vi "AlliGator Decay Fit Parameter Map Actions.vi"(0 "AlliGator Q Elements in":T6[](array[typedef]), 1 "VI in":refnum<vi>, 2 "Script in":bool, 5 "data value reference":refnum<data-value>, 7 "AlliGator Q Event in":T7=enum."GUI:Idle", 9 "Data":variant, 11 "error in (no error)":errorcluster) -> (3 "Script out":bool, 4 "AlliGator Q Elements out":T6[](array[typedef]), 6 "Data Value Reference out":refnum<data-value>, 10 "[Notebook Message]":T1[](array[typedef]) {"Message Style"."Font Size" min=6.0 step=1.0}, 15 "error out":errorcluster)   [LabVIEW 2021, in "AlliGator Action Engine.lvlib"]
doc: "Processes AlliGator decay fit parameter map-related actions."
uses:
  AlliGator Action Engine.lvlib
  Internal Variables/AlliGator Internal Variables v2.ctl
  <vilib>/vision/Image Controls.llb/IMAQ Image.ctl
  Internal Variables/AlliGator Gate Image Set.ctl
  Files/AlliGator FLI Dataset Type.ctl
  Files/AlliGator Data Series Type.ctl
  Dual-Channel Datasets/AlliGator Dataset Channel.ctl
  Settings/AlliGator Gate Arithmetic.ctl
  Source Image/AlliGator Displayed Image.ctl
  Image/Named ROI Description.ctl
  Phasor Graph/AlliGator Decay Metadata v3.ctl
  Decay Analysis/Decay Preprocessing/AlliGator Decay Background Subtraction Info.ctl
  Decay Analysis/Decay Preprocessing/AlliGator Baseline Subtraction Method.ctl
  Graphs/XY Graph/XY Graph Plot Shift Parameters.ctl
  Graphs/XY Graph/XY Graph Plot Shift Method.ctl
  Decay Analysis/Decay Preprocessing/AlliGator Decay Extrapolation Parameters.ctl
  Phasor/Calibration Phasor (m, phi).ctl
  Phasor/Phasor Reference Series.ctl
  Phasor/Phasor Calibration Map v2.ctl
  Phasor/Phasor (g, s).ctl
  Phasor Graph/AlliGator Raw Phasor Plot Data v5.ctl
  Phasor/Phasor Standard Deviation Options.ctl
  Phasor Plot/AlliGator Phasor Multi-Harmonic Data.ctl
  Phasor/Phasor Harmonic Data.ctl
  Decay Fit Parameter Map/AlliGator Decay Fit Options & Parameters v4.ctl
  Fits/IRF(X)PSED/Decay Fit Options v4.ctl
  Fits/Decay Convolution/Decay Model.ctl
  Fits/Residual Type.ctl
  Fits/IRF(X)PSED/Fit Weights Type v2.ctl
  Fits/Non-linear Fitting Method v2.ctl
  Fits/Fit Calculation Method.ctl
  Fits/Non-linear Fitting Algorithm.ctl
  Decay Analysis/Decay Fit/AlliGator Decay Fit Parameter Constraints 2.ctl
  Fits/IRF(X)PSED/Decay Fit Parameters In List.ctl
  Fits/IRF(X)PSED/MLE Baseline Offset Type.ctl
  Decay Analysis/Decay Preprocessing/AlliGator Decay Preprocessing Parameters.ctl
  Fits/IRF(X)PSED/Decay Fit Parameters & Derived Quantities List v2.ctl
  Fits/IRF(X)PSED/Decay Fit Result Constraint.ctl
  Decay Fit Parameter Map/AlliGator Parameter Maps Data.ctl
  AlliGator Q Event.ctl
  AlliGator Q Element.ctl
  Notebook/Notebook Message Object.ctl
  Rich Text Box/Text Formatting.ctl
  Rich Text Box/Text Colors.ctl
  Rich Text Box/Text Style.ctl
  Rich Text Box/Text Alignment.ctl
  Alligator Elements Order in Action Stack.ctl
  Globals, Variables, Constants/AlliGator Variables List.ctl
  GUI/AlliGator Image Display Type.ctl
  Palette/Image Palette Information.ctl
  Image/Image Display Palette Type.ctl
  Decay Fit Parameter Map/AlliGator Decay Parameter Map Update Event Data.ctl
  Rich Text Box/Text Format List.ctl
  GUI/AlliGator Windows List.ctl
  Utilities/Read-Write.ctl
  GUI/AlliGator Image Mouse Up Event Data.ctl
  Image/Image ROI Descriptor.ctl
  Image/Image Contour Definition.ctl
  Image/Image Contour ID.ctl
  Image/Image ROI Type.ctl
  Image/Image Control Refnum.ctl
  Files/Load-Save File Info.ctl
  Parameter Map/AlliGator New Parameter Map Set Event Data.ctl
  AlliGator Add Single Action to Stack.vi
  Variant/Variant to Data/Variant to [String].vi
  Variant/Variant to Data/Variant to String.vi
  <userlib>/_OpenG.lib/array/array.llb/Remove Duplicates from 1D Array (String)__ogtk.vi
  Variant/Variant to Data/Variant to I32.vi
  Variant/Variant to Data/Variant to Boolean.vi
  Local Decay Window/AlliGator Local Decay Window.lvlib
  Fits/Fits.lvlib
  Decay Fit Parameter Map/AlliGator Decay Fit Parameter Map.lvlib
  GUI/GUI.lvlib
  Variant/Variant to Data/Variant to Data.lvlib
  Globals, Variables, Constants/AlliGator Globals, Variables & Constants.lvlib
  Palette/Palette.lvlib
  GUI/AlliGator GUI.lvlib
  Image/Image.lvlib
  Files/Files.lvlib
  Sound/Sound.lvlib
  Source Image/AlliGator Source Image+.lvlib
  Parameter Map/AlliGator Parameter Map.lvlib
  Utilities/Utilities.lvlib
  Notebook/Notebook.lvlib
  <userlib>/_OpenG.lib/array/array.llb/openg_array.lvlib
  Phasor/Phasor.lvlib
  Decay Analysis/Decay Preprocessing/AlliGator Decay Preprocessing.lvlib
  Graphs/XY Graph/XY Graph Add-Ons.lvlib
  Phasor Graph/AlliGator Phasor Graph.lvlib
  Files/AlliGator Files.lvlib
  Internal Variables/AlliGator Internal Variables.lvlib
  Phasor Plot/AlliGator Phasor Plot.lvlib
  Decay Analysis/Decay Fit/AlliGator Decay Fit.lvlib
  Settings/AlliGator Settings+.lvlib
  Rich Text Box/Rich Text Box.lvlib
  Dual-Channel Datasets/AlliGator Dual-Channel Datasets.lvlib
panel:
  # "see the License on the block diagram (Ctrl+E or Window:Show Block Diagram)"
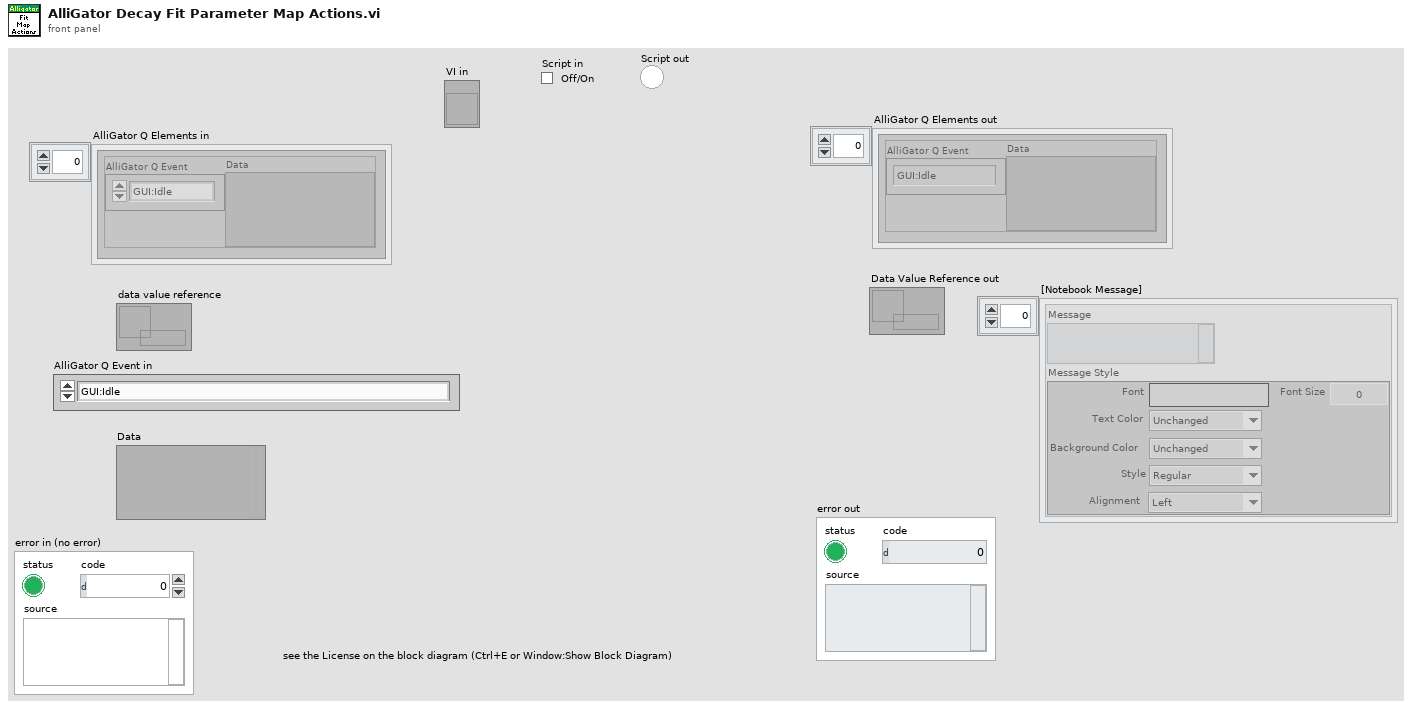
[diagram p1: front panel]
types:
  T1 = typedef "Notebook.lvlib/Notebook Message Object.ctl" = cluster{"Message":string, "Message Style":T2}
  T2 = typedef "Rich Text Box.lvlib/Text Formatting.ctl" = cluster{"Font":string, "Text Color":T3, "Background Color":T3, "Style":T4, "Font Size":dbl, "Alignment":T5}
  T3 = typedef "Rich Text Box.lvlib/Text Colors.ctl" = enum16{"Unchanged", "Black", "Blue", "Cyan", "Maroon", "Gray", "Violet", "Green", "Light Green", "Orange", "Yellow", "Magenta", "Red", "White"}
  T4 = typedef "Rich Text Box.lvlib/Text Style.ctl" = enum16{"Regular", "Bold", "Italic", "Underline", "Strikeout"}
  T5 = typedef "Rich Text Box.lvlib/Text Alignment.ctl" = enum16{"Left", "Right", "Center"}
  T6 = typedef "AlliGator Action Engine.lvlib/AlliGator Q Element.ctl" = cluster{"AlliGator Q Event":T7, "Data":variant}
  T7 = typedef "AlliGator Action Engine.lvlib/AlliGator Q Event.ctl" = enum16{"---- Files ----", "Files:Set Batch Export Files To Save", "Files:Set Dataset Loading & Pre-processing Options", "Files:Check #Frames in Dataset", "Files:Increment Frame Index", "Files:Open Mask Image", "Files:Open White Light Image", "Files:Open Single Dataset", "Files:New Folder of Folders Selected", "Files:Load File (all Types)_Scriptable", "Files:Move Flattened Series to Folders Series", "Files:Select Folder", "Files:Load FLI Dataset", "Files:Load Swiss SPAD 1 Dataset", "Files:Load Swiss SPAD 2 Dataset", "Files:Load .sdt FLI Dataset", "Files:Load .ptu FLI Dataset", "Files:Load .bin FLI Dataset", "Files:Load Single Gate Image Folder", "Files:Load I/m/phi Dataset (deprecated)", "Files:Load Single Image", "Files:Subtract Background File", "Files:Export FLI Dataset", "Files:Load HDF5 FLI Dataset", "Files:Set Destination File Path", "Files:Save Mask Image", "Files:Batch Conversion", "Files:New Folder Selected", "Files:Close FLI Dataset", "Files:Close FLI Dataset Series", "Files:Close White Light Image", "Files:Close Mask Image", "---- FLI Dataset ----", "FLI Dataset:Channel Arithmetic", "FLI Dataset:Export Average Lifetime Map as ASCII", "FLI Dataset:Export User-Defined Quantity Map as ASCII", "FLI Dataset:Python Function FLI Dataset Event", "FLI Dataset:ROI Analysis", "FLI Dataset:Tilted Logistic Square Gated IRF Characteristics Map", "FLI Dataset:Logistic Square Gated IRF Characteristics Map", "FLI Dataset:Square Gated IRF Characteristics Map", "FLI Dataset:Multi-ROI Single-Pixel Phasor Analysis", "FLI Dataset:Multi-ROI Single-Pixel NLSF Analysis", "FLI Dataset:All ROIs IRF Extraction", "FLI Dataset:All ROIs Decay Fit Non-Interactive (Fast + Individual IRF)", "FLI Dataset:All ROIs Phasor Analysis", "FLI Dataset:All ROIs Decay Fit", "FLI Dataset:Fluorescence Decay Statistics", "FLI Dataset:Update Decay Statistics Graph", "FLI Dataset:Get Decay from ROI", "FLI Dataset:All ROIs Average Lifetimes", "FLI Dataset:Save/Load Local IRFs", "FLI Dataset:Clear Local IRFs", "FLI Dataset:Phasor Calibration Maps (# Gates Series) Script", "FLI Dataset:Calibrated Phasor Map Series", "---- FLI Dataset Series ----", "FLI Dataset Series:Sum All Datasets in Series", "FLI Dataset Series:Add Dataset to Accumulated Dataset", "FLI Dataset Series:Display Accumulated Dataset", "FLI Dataset Series:Clear Dataset Series Sum", "FLI Dataset Series:Time-Series Analysis (NLSF)", "FLI Dataset Series:Time-Series Analysis (Phasor)", "---- Image ----", "Image:Update Image Profile Plots", "Image:Image Histogram Cursor Move", "Image:Image Histogram", "Image:Image Contrast", "Image:Set Image Histogram Cursor Move Flag", "Image:Clear Image Overlay", "Image:Use ROI as Search Area", "Image:Set ROI Diameter", "Image:Save Image Data as TIFF", "Image:Save Displayed Image with Overlay", "Image:Save Image Overlay Only", "Image:Save Image as Hot Pixel Mask", "Image:Change Source Image Color Palette", "Image:Copy Image to Clipboard", "Image:Source Image ROI Selection", "Image:Delete All ROIs", "Image:Delete All Unselected ROIs", "Image:Delete ROI", "Image:Merge All ROIs", "Image:Store ROI", "Image:Source Image ROI Storage", "Image:Export ROI Description to Notebook", "Image:Save ROI", "Image:Load ROI", "Image:Paste ROI Definition", "Image:Clear ROI", "Image:Identify ROIs in Mask Image", "Image:Create Complementary ROI", "Image:Create Contour ROI", "Image:Create ROI(s) from Pixels with Peak above Min_Scriptable", "Image:Create ROI(s) from Pixels with Intensity above Min_Scriptable", "Image:Compute ROI Statistics", "Image:Delete ROI(s) based on ROI Characteristics", "Image:Create ROI Grid", "Image:ROI to Individual Pixel ROIs", "Image:Python Function Source Image Event", "Image:Show Phasor Calibration Map ROI Centers", "Image:Convert ROI to Mask Image", "Image:Mouse Move", "Image:Mouse Up", "Image:Set Source Image Mouse Move Flag", "Image:Add Scale Bar Overlay", "Image:Delete Existing ROIs Option", "Image:Overlay ROI Median", "Image:Check Current ROI", "Image:Update True Pixel Value", "Image:Use ROI", "---- Decay ----", "Decay:Clear IRF/Reference Plot", "Decay:Add Decay to Graph", "Decay:Smoothen Plot", "Decay:Smoothen Plot Tail", "Decay:Average Selected Plots", "Decay:Extract IRF", "Decay:Optimal IRF Extraction", "Decay:Threshold IRF", "Decay:Fit to Model IRF", "Decay:Fit IRF to Square Gate", "Decay:Fit IRF to Logistic Square Gate", "Decay:Fit IRF to Tilted Logistic Square Gate", "Decay:Create Bounding Cursors Set", "Decay:Export Bounding Cursors Definition to Notebook", "Decay:Denoise Plot", "Decay:Compute Cumulative Function", "Decay:Use as Reference Decay", "Decay:Show Reference Decay/IRF", "Decay:Extrapolate Decay", "Decay:Create Head & Tail Bounding Cursors", "Decay:Store Cursor-defined Head & Tail Fractions", "Decay:Rebin Plot", "Decay:1-Normalize Decay", "Decay:[0-1]-Normalize Plot", "Decay:Straighten Decay", "Decay:Shift Decay", "Decay:Fold Decay", "Decay:Fit Decay", "Decay:Global Fit of Selected Decays", "Decay:Post Global Fit Script", "Decay:Add Global Fit Parameters to Graph", "Decay:Add Decay Parameter(s) to Plot (Graph)", "Decay:Export Decay to Phasor Graph", "Decay:Compute Average Lifetime", "Decay:Plot Convolution", "Decay:Graph Tip Strip Update", "---- Decay Statistics ----", "Decay Statistics:Tip Strip Update", "---- Intensity Time Trace ----", "Intensity Time Trace:Use File Timestamp", "Intensity Time Trace:Load Intensity Corrections File", "Intensity Time Trace:Clear Intensity Corrections File", "Intensity Time Trace:Tip Strip Update", "---- Phasor Plot ----", "Phasor Plot:Build Phasor Plot", "Phasor Plot:Change Phasor Plot Color Palette", "Phasor Plot:Adjust Phasor Plot Display Range", "Phasor Plot:Highlight Image ROI in Phasor Plot", "Phasor Plot:Save Phasor Plot Image with Overlay", "Phasor Plot:Export Complex Phasor Map", "Phasor Plot:Export Phasor Ratio Map", "Phasor Plot:Export Average Lifetime Map", "Phasor Plot:Compute Phase Lifetime Histogram", "Phasor Plot:Compute Phasor Ratio Histogram", "Phasor Plot:Compute Phase Lifetime vs Intensity Scatter Plot", "Phasor Plot:Weber 2-Component Decomposition", "Phasor Plot:Update Phasor Color Map Vertices", "Phasor Plot:Clear Phasor Overlay", "Phasor Plot:Use Segment Extremities as References", "Phasor Plot:Use UC/Segment Intersections as References", "Phasor Plot:Use UC/Principal Axis Intersections as References", "Phasor Plot:Use UC/Linear Fit Intersections as References", "Phasor Plot:Update Phasor Plot Reference", "Phasor Plot:Show Local Phasor Info in Phasor Plot", "Phasor Plot:Update Phasor Plot State", "Phasor Plot:Phasor Plot ROI Storage", "Phasor Plot:Phasor Plot ROI Selection", "Phasor Plot:Python Function Phasor Plot Event", "Phasor Plot:Overlay Phasor ROI, Ratio or Map in Source Image", "Phasor Plot:Compute Decay of Selected Phasors", "Phasor Plot:Phasor at Image Pixel", "Phasor Plot:Mouse Move", "Phasor Plot:Mouse Up", "Phasor Plot:Display Range Mouse Move", "Phasor Plot:Set Mouse Move Flag", "Phasor Plot:Update True Phasor Plot Value", "---- Phasor Graph ----", "Phasor Graph:Get Phasor Value", "Phasor Graph:Create New Phasor Plot Dialog", "Phasor Graph:Update Last Phasor Value", "Phasor Graph:Update Phasor (m, phi)", "Phasor Graph:Remove Single Phasor from Plot", "Phasor Graph:Add Single Phasor to Plot", "Phasor Graph:Remove Phasor Plot", "Phasor Graph:Remove Selected Phasor Plots", "Phasor Graph:Clear Phasor Data", "Phasor Graph:Clear Phasor Graph", "Phasor Graph:Cursor Move", "Phasor Graph:Draw Cursor Connecting Line", "Phasor Graph:Clear Cursor Connecting Line", "Phasor Graph:Find UC Intersection", "Phasor Graph:Use UC/Cursor-Defined Line Intersections", "Phasor Graph:Use Selected Plots Fitted Line/UC Intersections", "Phasor Graph:Use Selected Plots Principal Axis/UC Intersections", "Phasor Graph:Show Single Phasor", "Phasor Graph:Save Single Phasor Plot", "Phasor Graph:Save All Phasor Plots", "Phasor Graph:Load Phasor Plot(s)", "Phasor Graph:Phasor Multiplication", "Phasor Graph:Compute Average Phasor", "Phasor Graph:Compute Multiple Average Phasors (Selected Plots)", "Phasor Graph:Export Single Phasor Plot Phase Lifetimes", "Phasor Graph:Parameter 2 vs Parameter 1 Scatter Plot", "Phasor Graph:Use Cursor n Location", "Phasor Graph:Set Reference n to Current Phase Lifetime Value", "Phasor Graph:Set Reference n to Lifetime Value", "Phasor Graph:Set Cursor n Location", "Phasor Graph:Save Phasor Graph Image", "Phasor Graph:Update SEPL Plot", "Phasor Graph:Export Single Phasor Plot Data", "Phasor Graph:Export Selected Phasor Plots Data", "Phasor Graph:Python Function Phasor Graph Event", "Phasor Graph:Tip Strip Update", "---- Calibration ----", "Calibration:Set Calibration Type", "Calibration:Load/Save Phasor Calibration", "Calibration:Load/Save Phasor Calibration Series", "Calibration:Load/Save Phasor Calibration Map", "Calibration:Use as Calibration", "Calibration:Compute Optimal Calibration from Phasor References", "Calibration:Clear Phasor Calibration", "Calibration:Single Phasor Calibration Information", "Calibration:Use as Calibration Series", "Calibration:Use as Calibration Map", "Calibration:Clear Calibration Series", "Calibration:Phasor Calibration Series Information", "Calibration:Clear Calibration Map", "Calibration:Phasor Calibration Map Information", "Calibration:Apply Phasor Calibration", "Calibration:Update Single Plot Calibration", "Calibration:Update Multiple Plots Calibration", "Calibration:Clear Single Plot Calibration", "Calibration:Clear All Plots Calibrations", "Calibration:Clear Plot(s) Calibration(s)?", "---- Phasor Ratio ----", "Phasor Ratio:Clear Reference n", "Phasor Ratio:Toggle Selected Plot(s)  Lock to Reference 1", "Phasor Ratio:Use as Reference n", "Phasor Ratio:Send Reference n to Notebook", "Phasor Ratio:Toggle Selected Plot(s)  Lock to Reference 2", "Phasor Ratio:Compute Phasor Ratio at Mouse Location", "Phasor Ratio:Compute Phasor Plot's Average Phasor Ratio", "Phasor Ratio:Compute Time-Series Phasor Ratios", "Phasor Ratio:Fit Line to Phasor Ratio Plot", "Phasor Ratio:Save References", "Phasor Ratio:Load References", "Phasor Ratio:Update Phasor Reference 1", "Phasor Ratio:Update Phasor Reference 2", "Phasor Ratio:Move Cursor n to Reference n", "Phasor Ratio:Use as Phasor Reference 1 Lifetime", "Phasor Ratio:Use as Phasor Reference 2 Lifetime", "Phasor Ratio:Export Phasor Ratio Map as ASCII", "Phasor Ratio:Tip Strip Update", "---- Lifetime & Other Parameters Graph ----", "Lifetime:Compute Sliced Mean, SDV and CV Plots", "Lifetime:Plot Decay Shifts", "Lifetime:Plot Histogram", "---- Decay Fit Parameter Map ----", "Decay Fit Parameter Map:Export ROI NLSF Data as ASCII", "Decay Fit Parameter Map:Set Decay Fit Parameter Map Selection", "Decay Fit Parameter Map:Build Decay Fit Parameter Map", "Decay Fit Parameter Map:Change Decay Fit Parameter Map Color Palette", "Decay Fit Parameter Map:Export Decay Fit Parameter Map Data as ASCII", "Decay Fit Parameter Map:Export All Decay Fit Parameter Maps Data as ASCII", "Decay Fit Parameter Map:Selected Parameter Scatterplot", "Decay Fit Parameter Map:Parameter 2 vs Parameter 1 Scatterplot", "Decay Fit Parameter Map:Save Decay Fit Parameter Map Image", "Decay Fit Parameter Map:Save-Load IRFs & Fit Data", "Decay Fit Parameter Map:Update Local Decay Plots", "Decay Fit Parameter Map:Python Function Decay Fit Parameters Map Event", "Decay Fit Parameter Map:Overlay Decay Fit Parameter Map in Source Image", "Decay Fit Parameter Map:Selected Parameter vs Intensity Scatterplot", "Decay Fit Parameter Map:Mouse Up", "Decay Fit Parameter Map:Mouse Move", "Decay Fit Parameter Map:Display Range Mouse Move", "Decay Fit Parameter Map:Change Map Resolution", "Decay Fit Parameter Map:Variance Significance Maps", "Decay Fit Parameter Map:Fit Result Constraints Window", "Decay Fit Parameter Map:Use ROI", "---- Parameter Map ----", "Parameter Map:Export ROI Parameters Data as ASCII", "Parameter Map:Add Parameter Map Set", "Parameter Map:Delete Parameter Map Set", "Parameter Map:Update Parameter List", "Parameter Map:Build Parameter Map", "Parameter Map:Change Parameter Map Color Palette", "Parameter Map:Export Parameter Map Data as ASCII", "Parameter Map:Export All Parameter Maps Data as ASCII", "Parameter Map:Selected Parameter Scatterplot", "Parameter Map:Parameter 2 vs Parameter 1 Scatterplot", "Parameter Map:Selected Parameter vs Intensity Scatterplot", "Parameter Map:Save Parameter Map Image", "Parameter Map:Save-Load IRFs & Parameter Maps (TODO)", "Parameter Map:Set Parameter Map Selection", "Parameter Map:Python Function Parameter Map Event", "Parameter Map:Overlay Parameter Map in Source Image", "Parameter Map:Update Local Decay Plots", "Parameter Map:Mouse Up", "Parameter Map:Mouse Move", "Parameter Map:Display Range Mouse Move", "Parameter Map:Use ROI", "---- Generic Graph ----", "Generic Graph:Generic XY Graph Event", "Generic Graph:Python Function XY Graph Event", "Generic Graph:New Plot", "Generic Graph:Save Plot", "Generic Graph:XY Plot Histogram", "Generic Graph:Set XY Graph Plot Name", "Generic Graph:Set Last Cursor Style", "Generic Graph:Tip Strip Update", "---- GUI ----", "GUI:Start Script", "GUI:Type of Displayed Image Changed", "GUI:Gate Image Slide Changed", "GUI:Show Busy Icon", "GUI:Show Busy Icon & Abort Button", "GUI:Hide Busy Icon", "GUI:Hide Busy Icon & Abort Button", "GUI:Abort", "GUI:End Script", "GUI:Start Timing", "GUI:End Timing", "GUI:Set State Indicator", "GUI:Send Parameters JSON Strings to Clipboard", "GUI:Set Gate Step", "GUI:Idle", "GUI:Initialization", "GUI:Quit", "GUI:Increment Dataset Index", "GUI:Set Dataset Index to -1", "GUI:Time Series Slider Moved", "GUI:Time Series Slider Changed", "GUI:Toggle Playback or Loop", "GUI:Playback Script", "GUI:Set Phasor Frequency", "GUI:Open Window", "GUI:Start Test Script", "GUI:End Test Script", "GUI:Set Verbose Mode", "GUI:Set Verbose Settings Mode", "GUI:Initialize Python Session", "DEBUG"}
  T8 = typedef "AlliGator Decay Fit Parameter Map.lvlib/AlliGator Decay Fit Parameter Map Control Refnums.ctl" = cluster{"Decay Fit Parameter Map Color Scale":refnum<vi>, "Decay Fit Parameter":refnum<vi>, "Max Parameter":refnum<vi>, "Min Parameter":refnum<vi>, "Decay Fit Parameter Map Display":refnum<vi>, "Decay Fit Parameter Map Display Range":refnum<vi>, "Decay Parameter Map X":refnum<vi>, "Decay Parameter Map Y":refnum<vi>, "Decay Parameter Map Value":refnum<vi>}
  T9 = typedef "AlliGator GUI.lvlib/AlliGator Dataset Ctrl Refnums.ctl" = cluster{"Current Data":refnum<vi>, "Gate Image Slide":refnum<vi>, "Time Point Slide":refnum<vi>, "Current Time Stamp":refnum<vi>, "Save Image":refnum<vi>, "Displayed Image":refnum<vi>, "Phasor Overlay Color":refnum<vi>, "Image Color Scale":refnum<vi>, "Use ROI as Search Area":refnum<vi>, "Source Image ROI Color":refnum<vi>, "True Pixel Value":refnum<vi>, "Source Image Display":refnum<vi>, "CPU":refnum<vi>}
  T10 = typedef "AlliGator Action Engine.lvlib/Alligator Elements Order in Action Stack.ctl" = enum16{"Enqueue 2 AFTER 1", "Enqueue 2 BEFORE 1"}
  T11 = typedef "AlliGator Source Image+.lvlib/AlliGator Image Display Type.ctl" = enum16{"Source Image", "Phasor Plot", "Decay Fit Parameter Map", "Parameter Map"}
  T12 = typedef "AlliGator Globals, Variables & Constants.lvlib/AlliGator Variables List.ctl" = enum16{"---- GUI ----", "GUI:Initialization Status", "GUI:State Indicators Refnum", "GUI:Original AlliGator Menu Items", "GUI:Current Action Loop State", "GUI:Script in progress", "GUI:Playback", "GUI:Loop Playback", "GUI:Search ROI Used", "GUI:Search ROI", "Image Histogram Max Legend Size", "Decay Graph Max Legend Size", "Intensity Graph Max Legend Size", "Decay Statistics Graph Max Legend Size", "Phasor Graph Max Legend Size", "Phasor Ratio Graph Max Legend Size", "Lifetime Graph Max Legend Size", "---- Files ----", "Files:Export Dataset Frames as Individual Files", "Files:Show Batch Export Help Balloons", "Files:Frames in Dataset", "Files:ptu File Frame Start Indices", "Files:Current Frame in Dataset", "Files:Current Frame Timestamp", "Files:Dataset Loaded", "Files:Dataset Metadata", "Files:Dataset Channel", "Files:Dataset Data Description", "Files:Background Dataset Metadata", "Files:Background Dataset Channel", "Files:Background Dataset Data Description", "Files:Background File Subtraction", "Files:Background File Path", "Files:Background File Pile-up Correction", "Files:Background File Pixel Well Capacity", "Files:Background File Scaling Factor", "Files:Current Dataset Load Settings", "Files:Dataset Path", "Files:ICCD-specific Information", "Files:Macrotime Gate Separation", "------ Python Plugins ------", "Python Plugins:Information", "Python Plugins:Python Session", "Python Plugins:Valid Python Session?", "---- Source Image ----", "Source Image:ROIs", "Source Image:Current ROI", "Source Image:ROI Event Refnum", "X_Source Image:Display Range", "X_Source Image:Palette Information", "X_Source Image:Type of Displayed Image", "X_Time Gate Slider", "Source Image:Palette List", "Source Image:Scale", "Source Image:ROI Overlay Color", "Source Image:Overlay to Erase", "Source Image:Is Displayed Image Accumulated", "Source Image:White Light Image Modified", "Source Image:Mask Image Modified", "---- Image Profile Window ----", "Image Profile:Window Event Refnum", "Image Profile:IntensityType", "Image Profile:Intensity Average Type", "Image Profile:Intensity-weighted SDV", "Image Profile:Box Profile Type", "Image Profile:Window Open", "Image Profile:Plotted Fit Parameter", "------ Phasor Graph -------", "Phasor Graph:Show Line", "---- Phasor Plot ---", "Phasor Plot:Parameters Changed", "Phasor Plot:FLI Dataset Modified since last Calculation", "Phasor Harmonics Data", "Selected Phasor Harmonics", "Phasor Harmonic Manager Event Refnum", "Phasor Plot:ROIs", "Phasor Plot:Current ROI", "Phasor Plot:ROI Event Refnum", "Phasor Plot:Image Reference Points", "Phasor Plot:Computed", "Phasor Plot:Palette Information", "Phasor Plot:Palette List", "Phasor Plot:Phasor Ratio Palette Information", "Phasor Plot:Phasor Ratio Palette List", "Phasor Plot:Image Scale", "Phasor Plot:Image Overlay to Erase", "Phasor Plot:Image Elements to Update", "Phasor Plot:Current Calculation Parameters", "Phasor Plot:Current Calibration Options", "Phasor Plot:Reset Cumulated Phasor Plot", "Phasor Plot:Reference 1", "Phasor Plot:Lifetime Reference 1", "Phasor Plot:Reference 1 Frequency", "Phasor Plot:Reference 2", "Phasor Plot:Lifetime Reference 2", "Phasor Plot:Reference 2 Frequency", "---- Decay Analysis ----", "Number of Selected Decays to Fit", "LS Fit Results", "LAR Fit Results", "BS Fit Results", "Last Decay Max - Min", "Best Fit Parameters", "Best Fit Parameter Names", "Actual Size X", "Actual Size Y", "Binning X", "Binning Y", "Actual # Gates", "Dataset Number", "Gates to...", "Gates Skipped", "Gates to keep", "Gate Step", "Gate Separation", "Reversed Gates", "Pile-up Correction", "Pixel Well Capacity", "Background Subtracted", "Background Subtraction Method", "Background Definition Range", "Background File (deprecated)", "Number of Dataset Accumulated", "Array of Accumulated Dataset Paths", "Do Averaged Datasets", "Destination File Path", "Process Plot Target", "Use 1/D as Phasor Frequency", "---- Decay Fit Parameter Map -----", "Decay Fit Parameter Map:Palette Information", "Decay Fit Parameter Map:Palette List", "Decay Fit Parameter Map:X Resolution", "Decay Fit Parameter Map:Y Resolution", "Decay Fit Parameter Map:Use Decay Fit Result Constraints", "Decay Fit Parameter Map:Decay Fit Result Constraints", "Decay Fit Parameter Map:Decay Fit Result Constraints Applied", "---- Parameter Map ----", "Parameter Map:Palette Information", "Parameter Map:Palette List", "------- Local Decay Window ---------", "Local Decay Graph Window:Event Refnum", "Local Decay Graph Window:Use normalized IRF for convolution", "----- Miscellaneous ----", "Misc:Skippable Dialog Windows Status"}
  T13 = typedef "Palette.lvlib/Image Palette Information.ctl" = cluster{"Palette Name [# Colors,int?,inv?]":string, "Palette Type":T14, "Palette Colors":u32[], "Interpolate?":bool}
  T14 = typedef "Image.lvlib/Image Display Palette Type.ctl" = u32
  T15 = typedef "Notebook.lvlib/Text Format List.ctl" = enum16{"Message", "Result", "Error", "Setting", "Verbose", "Warning"}
  T16 = typedef "AlliGator Decay Fit Parameter Map.lvlib/AlliGator Decay Parameter Map Update Event Data.ctl" = cluster{"Parameter":T17, "Parameter changed":bool}
  T17 = typedef "Fits.lvlib/Decay Fit Parameters & Derived Quantities List v2.ctl" = enum16{"Offset", "Baseline", "A_1", "tau_1", "A_2", "tau_2", "<tau>_a", "f1_a", "f2_a", "<tau>_i", "f1_i", "f2_i", "-", "R^2", "Chi^2"}
  T18 = typedef "AlliGator GUI.lvlib/AlliGator Windows List.ctl" = enum16{"AlliGator Window", "Settings Window", "Notebook Window", "Dataset Information Window", "Source Image ROI Manager Window", "Phasor Plot ROI Manager Window", "Phasor Harmonic Manager Window", "Histogram Window", "Image Profile Window", "Local Decay Window", "About Window", "Batch Conversion Window", "Shot Noise Influence on Average Lifetime", "Fit Method Benchmark", "Camera Noise Influence on Lifetime", "AlliGator Alias Definition", "Fit Result Constraints Window"}
  T19 = typedef "Utilities.lvlib/Read-Write.ctl" = enum16{"Read", "Write"}
  T20 = typedef "AlliGator GUI.lvlib/AlliGator Image Mouse Up Event Data.ctl" = cluster{"Current ROI Tool":u32, "ROI Descriptor":T21, "Shift":bool, "Alt":bool, "Image Display Refnum":T25}
  T21 = typedef "Image.lvlib/Image ROI Descriptor.ctl" = cluster{"Global Rectangle":i32[], "Contours":T22[]}
  T22 = typedef "Image.lvlib/Image Contour Definition.ctl" = cluster{"Contour Type":T23, "ROI Type":T24, "Points":i32[]}
  T23 = typedef "Image.lvlib/Image Contour ID.ctl" = enum32{"External", "Internal"}
  T24 = typedef "Image.lvlib/Image ROI Type.ctl" = enum16{"No Selection", "Point", "Line", "Rectangle", "Oval", "Polygon", "Freehand Region", "Annulus", "Unused2", "Unused3", "Broken Line", "Freehand Line", "Rotated Rectangle"}
  T25 = typedef "Image.lvlib/Image Control Refnum.ctl" = refnum<vi>
  T26 = cluster{"Fit Parameter 1":T17, "Fit Parameter 2":T17}
  T27 = typedef "Files.lvlib/Load-Save File Info.ctl" = cluster{"Load/Save":bool, "File Path":path}
  T28 = typedef "AlliGator Parameter Map.lvlib/AlliGator New Parameter Map Set Event Data.ctl" = cluster{"New Parameter Set Name":string, "Parameter Map Names":string[]}
  T29 = typedef "Fits.lvlib/Decay Fit Parameters & Derived Quantities List.ctl" = enum16{"Offset", "Baseline", "A_1", "tau_1", "A_2", "tau_2", "<tau>_a", "f1_a", "f2_a", "<tau>_i", "f1_i", "f2_i", "-", "R^2", "Chi^2"}
  T30 = typedef "ROI Descriptor" = cluster{"Global Rectangle":i32[], "Contours":cluster{"ID":enum32{"External", "Internal"}, "Type":u32, "Coordinates":i32[]}[]}
  T31 = typedef "AlliGator Decay Fit Parameter Map.lvlib/AlliGator Function Parameters.ctl" = cluster{"Function":T32, "Amplitude":dbl, "Exponent/Scale":dbl, "Baseline":dbl, "Residuals SDV":dbl, "Minimum CL (%)":dbl, "Analysis Type":enum32{"Reference", "New Sample"}, "Bootstrap SDV x Scale Factor":dbl, "Residuals SDV x Scale Factor":dbl, "Low CL Percentile to Reject (%)":dbl}
  T32 = typedef "AlliGator Lifetime & Other Parameters.lvlib/AlliGator CV(tau) Model Function.ctl" = enum16{"Single-Exponential", "Power Law"}
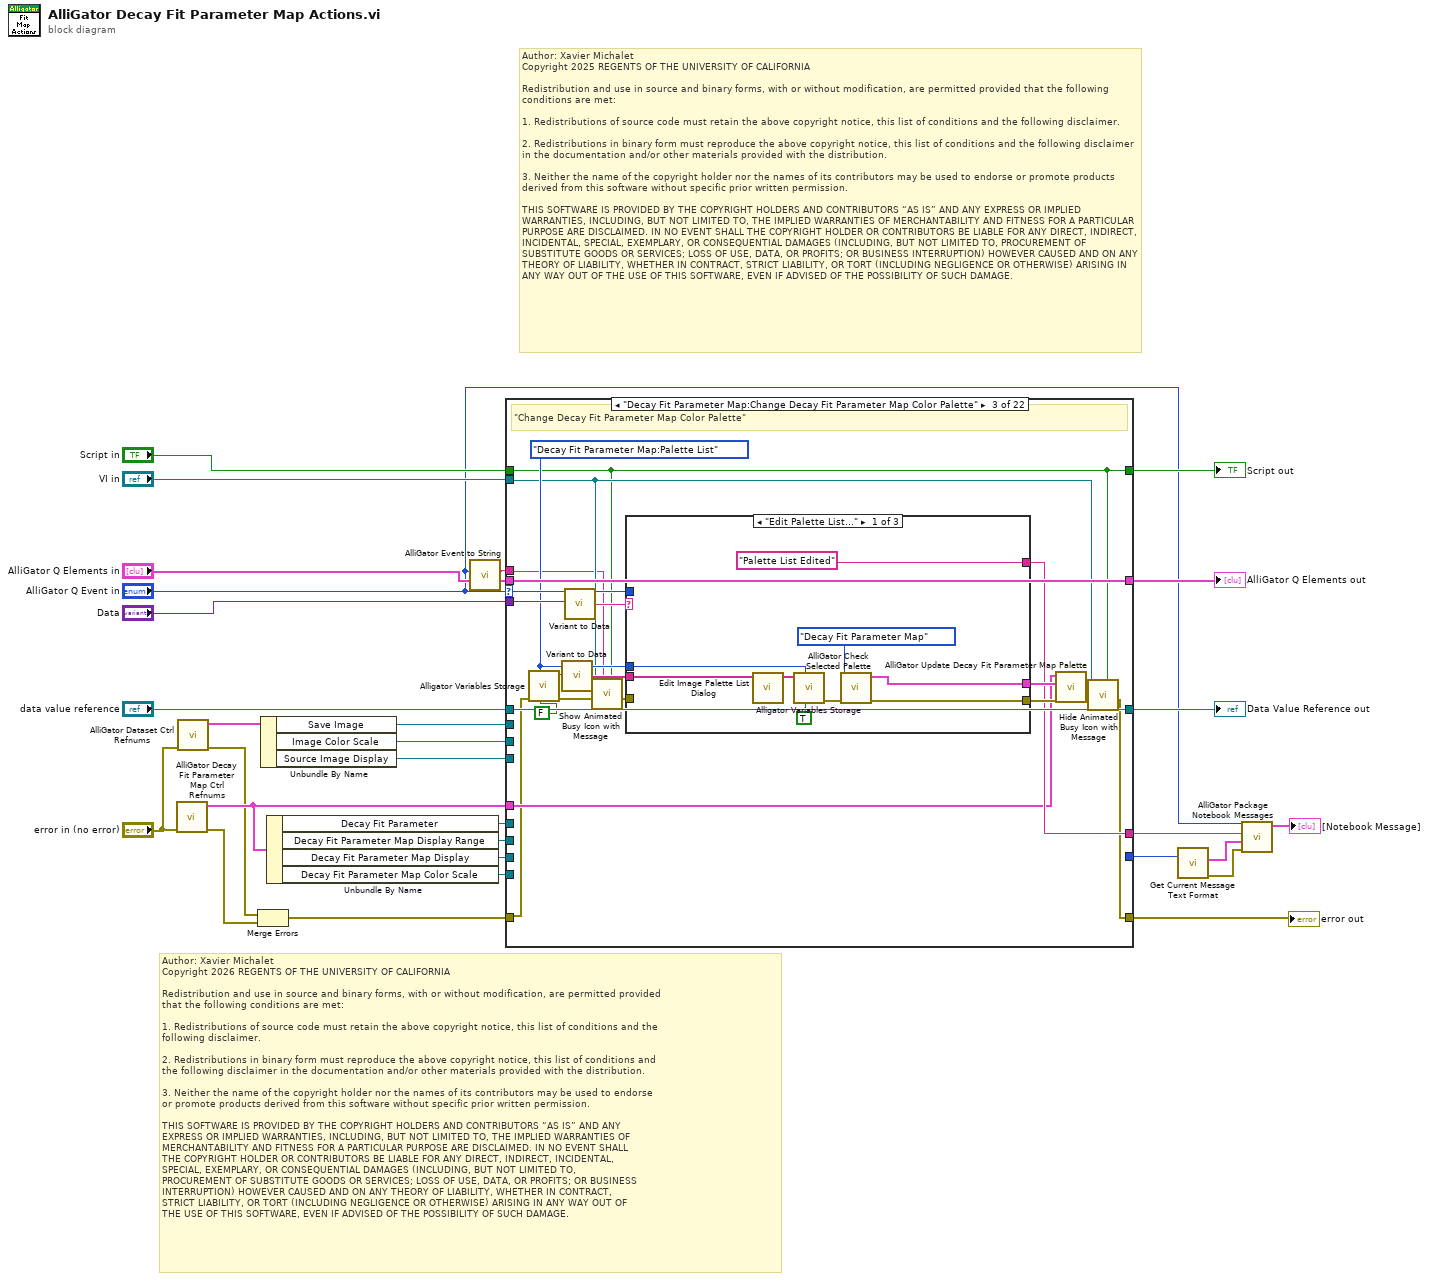
[diagram p0: block diagram]
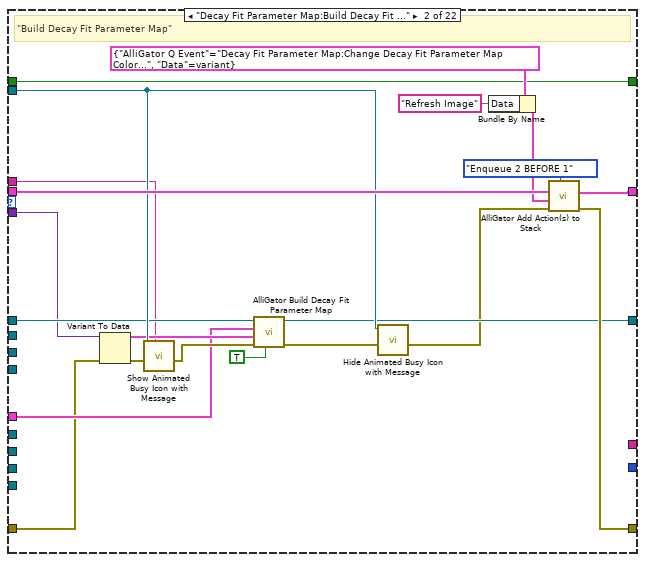
[diagram p3: hidden frame]
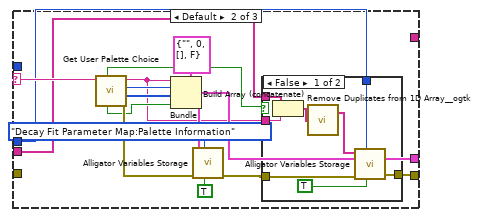
[diagram p4: hidden frame]
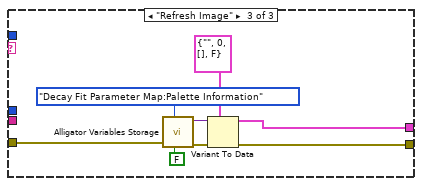
[diagram p6: hidden frame]
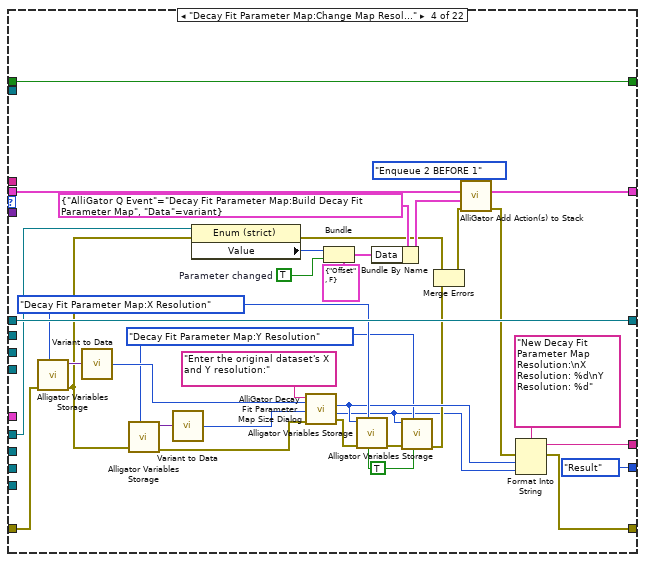
[diagram p7: hidden frame]
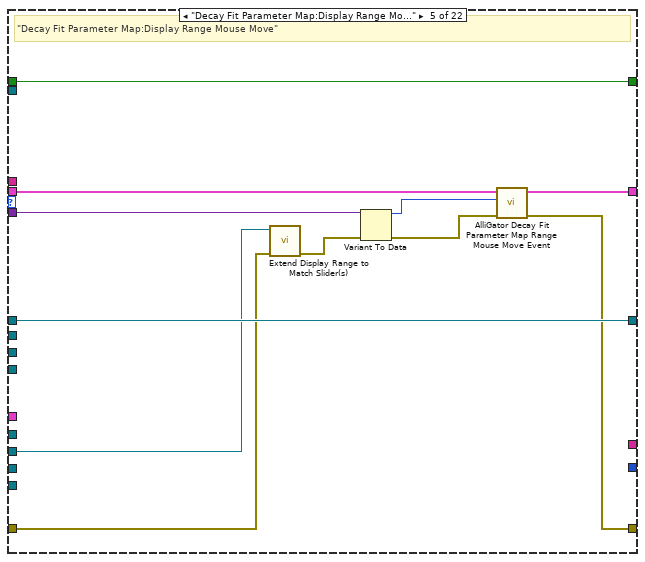
[diagram p8: hidden frame]
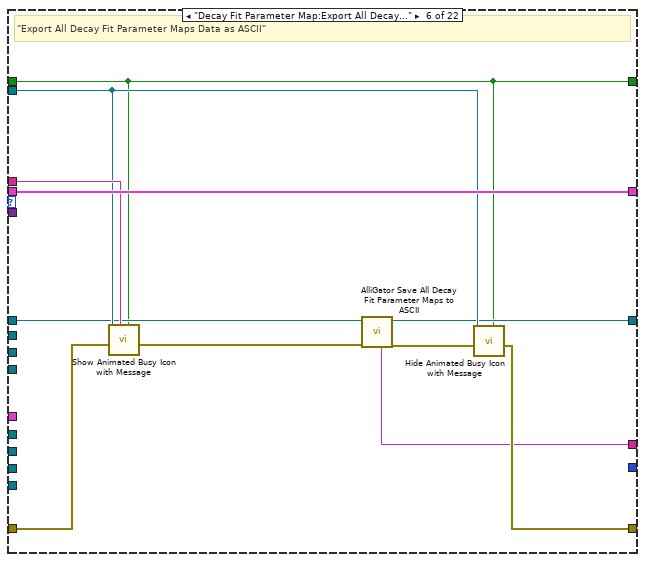
[diagram p9: hidden frame]
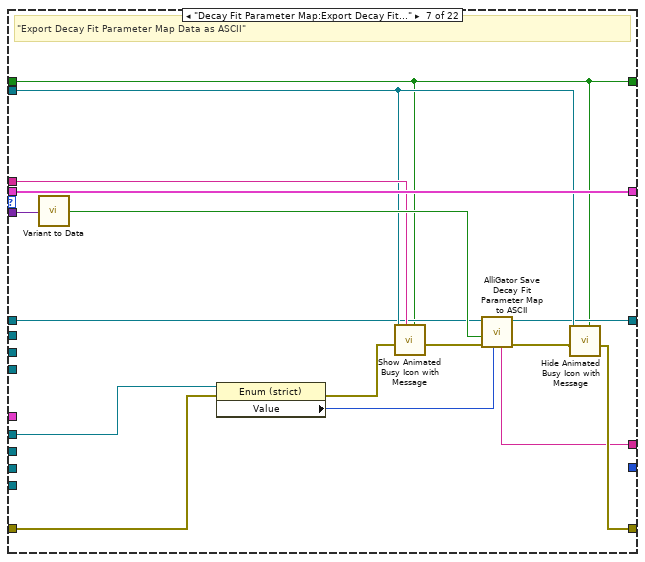
[diagram p10: hidden frame]
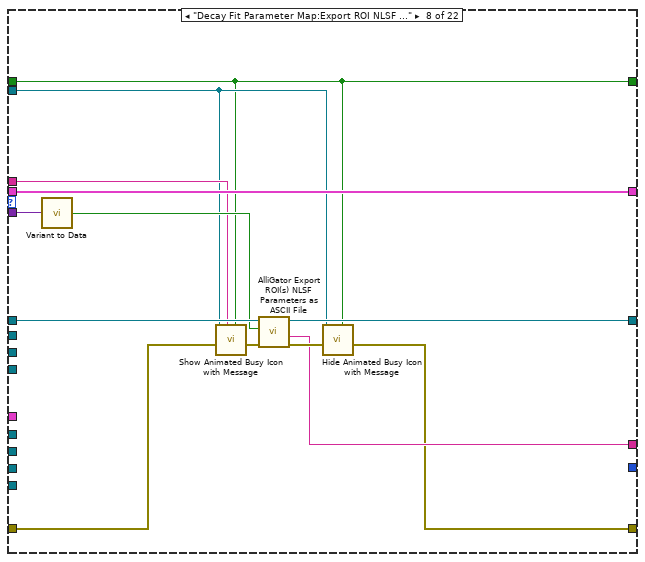
[diagram p11: hidden frame]
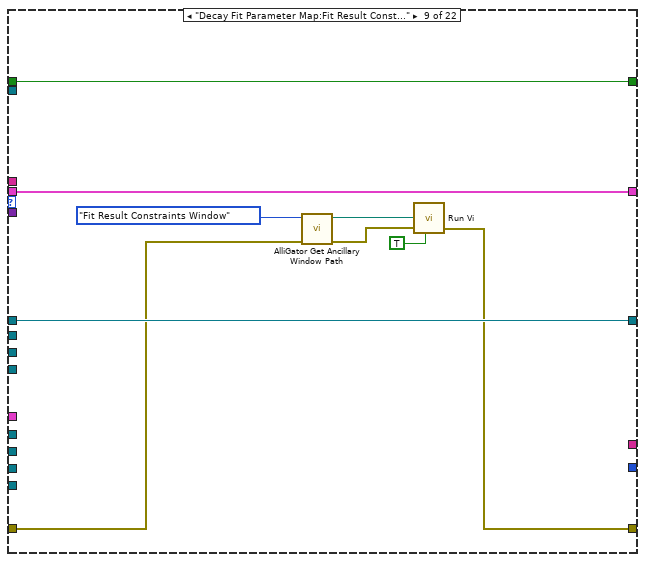
[diagram p12: hidden frame]
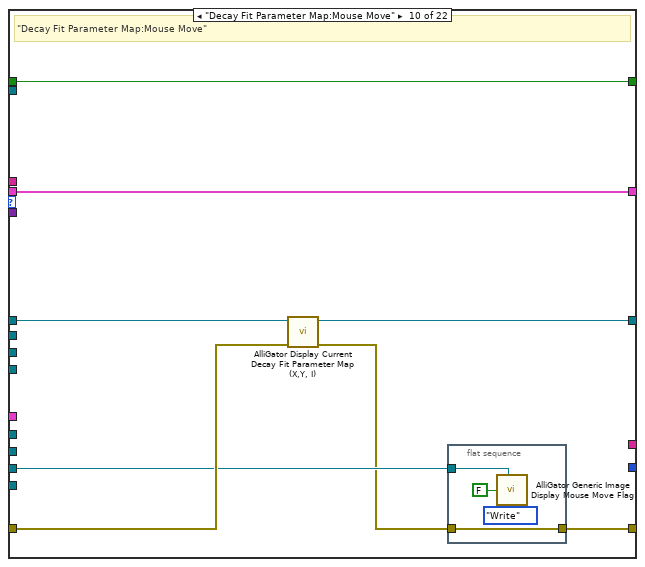
[diagram p13: hidden frame]
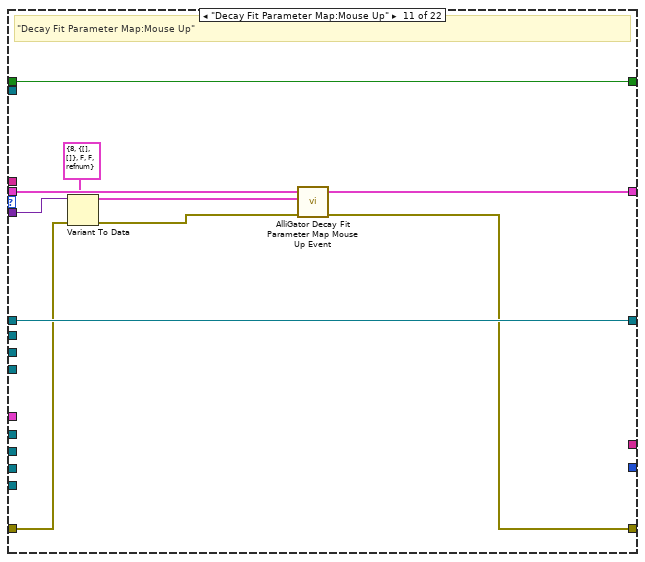
[diagram p14: hidden frame]
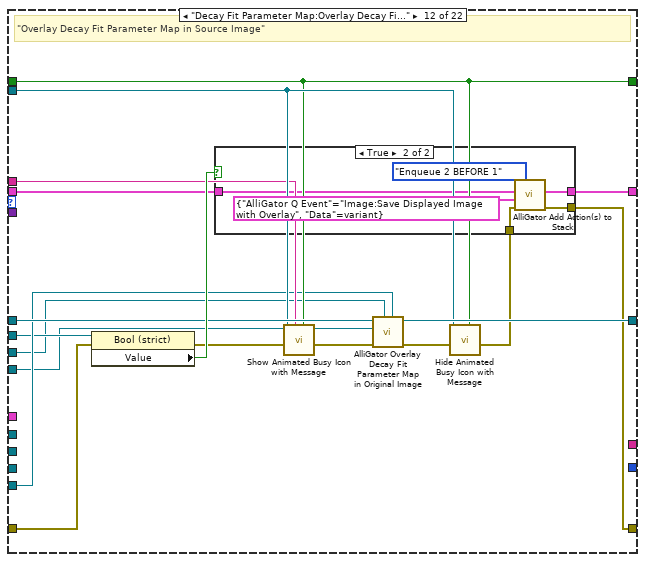
[diagram p15: hidden frame]
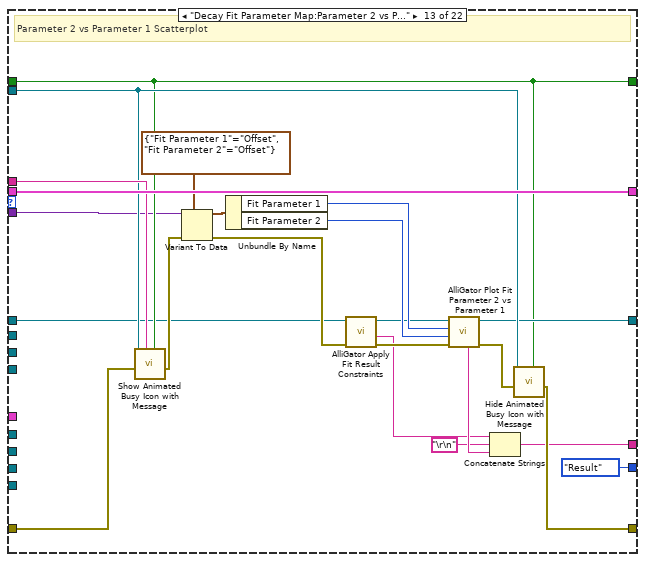
[diagram p17: hidden frame]
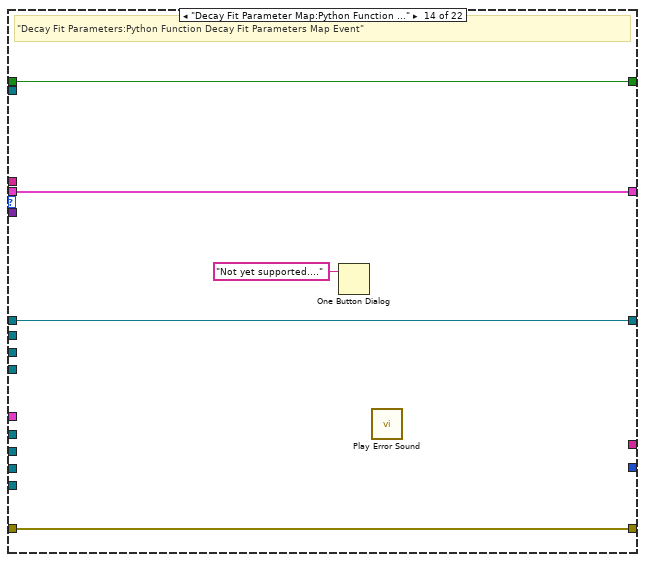
[diagram p18: hidden frame]
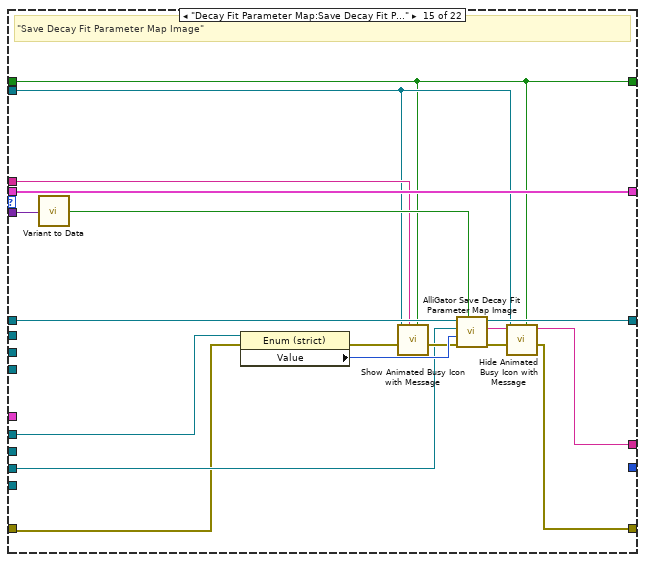
[diagram p19: hidden frame]
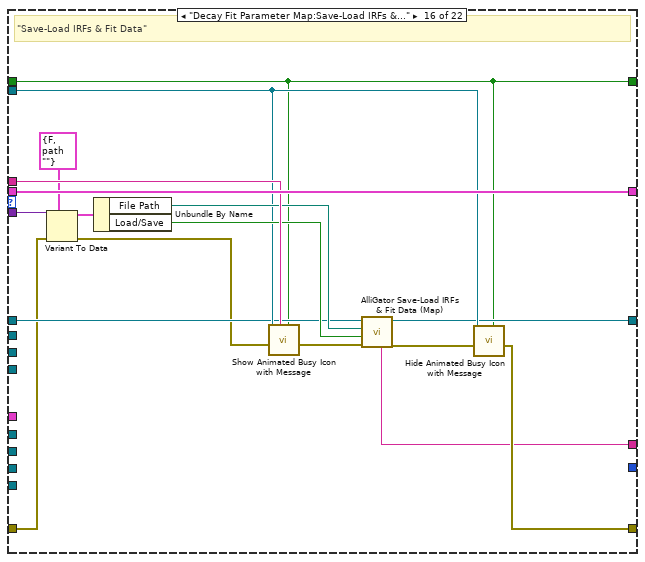
[diagram p20: hidden frame]
diagram:
  # "Author: Xavier Michalet\nCopyright 2026 REGENTS OF THE UNIVERSITY OF CALIFORNIA\n\nRedistribution and use in source and binary forms, with or without modification, are permitted provided\nthat the following conditions are met:\n\n1. Redistributions of source code must retain the above copyright notice, this list of conditions and the\nfollowing disclaimer.\n\n2. Redistributions in binary form must reproduce the above copyright notice, this list of conditions and\nthe following disclaimer in the documentation and/or other materials provided with the distribution.\n\n3. Neither the name of the copyright holder nor the names of its contributors may be used to endorse \nor promote products derived from this software without specific prior written permission.\n\nTHIS SOFTWARE IS PROVIDED BY THE COPYRIGHT HOLDERS AND CONTRIBUTORS “AS IS” AND ANY \nEXPRESS OR IMPLIED WARRANTIES, INCLUDING, BUT NOT LIMITED TO, THE IMPLIED WARRANTIES OF\nMERCHANTABILITY AND FITNESS FOR A PARTICULAR PURPOSE ARE DISCLAIMED. IN NO EVENT SHALL\nTHE COPYRIGHT HOLDER OR CONTRIBUTORS BE LIABLE FOR ANY DIRECT, INDIRECT, INCIDENTAL, \nSPECIAL, EXEMPLARY, OR CONSEQUENTIAL DAMAGES (INCLUDING, BUT NOT LIMITED TO, \nPROCUREMENT OF SUBSTITUTE GOODS OR SERVICES; LOSS OF USE, DATA, OR PROFITS; OR BUSINESS\nINTERRUPTION) HOWEVER CAUSED AND ON ANY THEORY OF LIABILITY, WHETHER IN CONTRACT, \nSTRICT LIABILITY, OR TORT (INCLUDING NEGLIGENCE OR OTHERWISE) ARISING IN ANY WAY OUT OF\nTHE USE OF THIS SOFTWARE, EVEN IF ADVISED OF THE POSSIBILITY OF SUCH DAMAGE."
  # "Author: Xavier Michalet\nCopyright 2025 REGENTS OF THE UNIVERSITY OF CALIFORNIA\n\nRedistribution and use in source and binary forms, with or without modification, are permitted provided that the following conditions are met:\n\n1. Redistributions of source code must retain the above copyright notice, this list of conditions and the following disclaimer.\n\n2. Redistributions in binary form must reproduce the above copyright notice, this list of conditions and the following disclaimer in the documentation and/or other materials provided with the distribution.\n\n3. Neither the name of the copyright holder nor the names of its contributors may be used to endorse or promote products derived from this software without specific prior written permission.\n\nTHIS SOFTWARE IS PROVIDED BY THE COPYRIGHT HOLDERS AND CONTRIBUTORS “AS IS” AND ANY EXPRESS OR IMPLIED WARRANTIES, INCLUDING, BUT NOT LIMITED TO, THE IMPLIED WARRANTIES OF MERCHANTABILITY AND FITNESS FOR A PARTICULAR PURPOSE ARE DISCLAIMED. IN NO EVENT SHALL THE COPYRIGHT HOLDER OR CONTRIBUTORS BE LIABLE FOR ANY DIRECT, INDIRECT, INCIDENTAL, SPECIAL, EXEMPLARY, OR CONSEQUENTIAL DAMAGES (INCLUDING, BUT NOT LIMITED TO, PROCUREMENT OF SUBSTITUTE GOODS OR SERVICES; LOSS OF USE, DATA, OR PROFITS; OR BUSINESS INTERRUPTION) HOWEVER CAUSED AND ON ANY THEORY OF LIABILITY, WHETHER IN CONTRACT, STRICT LIABILITY, OR TORT (INCLUDING NEGLIGENCE OR OTHERWISE) ARISING IN ANY WAY OUT OF THE USE OF THIS SOFTWARE, EVEN IF ADVISED OF THE POSSIBILITY OF SUCH DAMAGE."
  n1 = call "AlliGator Decay Fit Parameter Map Ctrl Refnums.vi"("error in (no error)"="error in (no error)") -> ("error out"=w1:errorcluster, "Decay Fit Map Ctrl Refums"=w13:T8)  [unwired: 9 in]
  n2 = call "AlliGator Dataset Ctrl Refnums.vi"("error in (no error)"="error in (no error)") -> ("error out"=w3:errorcluster, "Dataset Control References"=w8:T9)  [unwired: 9 in]
  n3 = Merge Errors(w3, w1) -> (w2:errorcluster)
  n4 = Unbundle By Name(w8) -> ("Save Image"=w7:refnum<vi>, "Image Color Scale"=w6:refnum<vi>, "Source Image Display"=w5:refnum<vi>)
  n5 = Unbundle By Name(w13) -> ("Decay Fit Parameter"=w12:refnum<vi>, "Decay Fit Parameter Map Display Range"=w11:refnum<vi>, "Decay Fit Parameter Map Display"=w10:refnum<vi>, "Decay Fit Parameter Map Color Scale"=w9:refnum<vi>)
  n6 = call "AlliGator Event to String.vi"("AlliGator Q Event"="AlliGator Q Event in") -> ("String"=w22:string)  [unwired: 8 in]
  n7 = case shown="\"Decay Fit Parameter Map:Change Decay Fit Parameter Map Color Palette\"" "AlliGator Q Event in" {
    selector: "AlliGator Q Event in" -> [_ _ w74 _ _ _ _ _ _ _ _ _ _ _ _ _ _ _ _ _ _ _]
    tunnel: "Data" -> [_ w40 w75 _ w157 _ w188 w201 _ _ w228 _ w275 _ w303 w318 w339 w361 w376 w389 _ w434]
    tunnel: "AlliGator Q Elements in" -> [w33 w54 w71 w142 w160 w173 w189 w202 w211 w219 w231 w246 w282 w287 w304 w321 w342 w364 w377 w390 w404 w439]
    tunnel: [w33 w53 w71 w141 w159 w173 w189 w202 w211 w219 w230 w245 w282 w287 w304 w321 w342 w364 w377 w390 w403 w439] -> w24
    tunnel: "VI in" -> [_ w45 w59 _ _ w170 w183 w192 _ _ _ w244 w279 _ w292 w313 w337 w359 _ w381 w394 _]
    tunnel: "Script in" -> [w30 w37 w58 w150 w161 w165 w178 w191 w209 w218 w232 w243 w276 w283 w291 w308 w333 w355 w367 w380 w393 w437]
    tunnel: w22 -> [_ w38 w57 _ _ w171 w185 w194 _ _ _ w242 w280 _ w294 w319 w340 w362 _ w379 w392 _]
    tunnel: w2 -> [w32 w34 w55 w143 w154 w163 w174 w190 w204 w217 w224 w236 w260 w286 w288 w305 _ w343 w365 w378 w396 w433]
    tunnel: [w32 w47 w60 w132 w158 w172 w186 w193 w203 w212 w229 w239 w281 w286 w293 w320 w341 w363 w368 w382 w395 w432] -> w14
    tunnel: "data value reference" -> [w31 w44 w69 w151 w162 w168 w181 w200 w210 w216 w233 w248 w266 w285 w302 w311 w329 w352 w370 w387 w405 w438]
    tunnel: [w31 w43 w69 w151 w162 w169 w182 w199 w210 w215 w233 w247 w278 w285 w301 w312 w335 w357 w370 w386 w401 w438] -> w29
    tunnel: [_ _ w67 w130 _ w164 w177 w196 _ _ _ _ w264 _ w300 w307 w326 w348 w369 _ w402 _] -> w19
    tunnel: [w30 w37 w58 w150 w161 w165 w178 w191 w209 w218 w232 w243 w276 w283 w291 w308 w333 w355 w367 w380 w393 w437] -> w21
    tunnel: [_ _ _ Text_Format_List."Result" ("Text Format") _ _ _ _ _ _ _ _ Text_Format_List."Result" ("Text Format") _ _ _ Text_Format_List."Result" ("Text Format") Text_Format_List."Result" ("Text Format") _ _ Text_Format_List."Result" ("Text Format") _] -> w16
    tunnel: w13 -> [_ w35 w56 _ _ _ _ _ _ _ _ _ _ _ _ _ _ _ _ _ _ _]
    tunnel: w12 -> [_ _ _ w120 _ _ w175 _ _ _ _ _ _ _ w289 _ w322 w344 w366 _ w391 _]
    tunnel: w11 -> [_ _ _ _ w152 _ _ _ _ _ _ _ _ _ _ _ _ _ _ _ _ _]
    tunnel: w10 -> [_ _ _ _ _ _ _ _ _ w214 _ _ _ _ w290 _ _ _ _ _ _ w430]
    tunnel: w9 -> [_ _ _ _ _ _ _ _ _ _ _ w238 _ _ _ _ _ _ _ _ _ _]
    tunnel: w7 -> [_ _ _ _ _ _ _ _ _ _ _ w237 _ _ _ _ _ _ _ _ _ _]
    tunnel: w6 -> [_ _ _ _ _ _ _ _ _ _ _ w235 _ _ _ _ _ _ _ _ _ _]
    tunnel: w5 -> [_ _ _ _ _ _ _ _ _ _ _ w234 _ _ _ _ _ _ _ _ _ _]
    frame "---- Decay Fit Parameter Map ----", Default {
    }
    frame "Decay Fit Parameter Map:Build Decay Fit Parameter Map" {
      # "\"Build Decay Fit Parameter Map\""
      n8 = Variant To Data(error in=w34, Variant=w40) -> (data=w41:T16, error out=w39:errorcluster)  [unwired: 1 in]
      n9 = call "Show Animated Busy Icon with Message.vi"("Message"=w38, "Error In"=w39, "Target VI Refnum"=w45) -> ("Error Out"=w46:errorcluster)  [unwired: 8 in]
      n10 = call "AlliGator Build Decay Fit Parameter Map.vi"("Compute Decay Fit Parameter Map (T)"=TRUE, "error in (no error)"=w46, "Decay Fit Parameter Map Update Event Data"=w41, "Decay Fit Map Ctrl Refums"=w35, "AlliGator Internal Variables DVR"=w44) -> ("error out"=w52:errorcluster, "AlliGator Internal Variables DVR"=w43:refnum<data-value>)  [unwired: 1 in, 4 out]
      n11 = call "Hide Animated Busy Icon with Message.vi"("Error In"=w52, "Target VI reference"=w45) -> ("Error Out"=w42:errorcluster)  [unwired: 9 in]
      n12 = Bundle By Name(cluster=T6 {"AlliGator Q Event"=enum."Decay Fit Parameter Map:Change Decay Fit Parameter Map Color Palette", "Data"=variant} ("Alligator Atomic Action"), "Data"="Refresh Image") -> (w48:T6)
      n13 = call-poly "AlliGator Add Action(s) to Stack.vi"("Elements Order in Action Stack (Default: 2 BEFORE 1)"=Alligator_Elements_Order_in_Action_Stack."Enqueue 2 BEFORE 1", "Error In"=w42, "Alligator Atomic Action"=w48, "Alligator Queue Element 1"=w54) -> ("Error Out"=w47:errorcluster, "Alligator Queue Element 1 (+ 2)"=w53:T6[])  [unwired: 6 in]
    }
    frame "Decay Fit Parameter Map:Change Decay Fit Parameter Map Color Palette" {
      w63 = AlliGator_Variables_List."Decay Fit Parameter Map:Palette List" ("Alligator Variable")
      # "\"Change Decay Fit Parameter Map Color Palette\""
      n14 = call "Alligator Variables Storage.vi"("Get(F)/Set"=FALSE, "AlliGator Variable"=w63, "Error In"=w55) -> ("Error Out"=w62:errorcluster, "Data out"=w66:variant)  [unwired: 6 in, 1 out]
      n15 = call-poly "Variant to Data.vi"("Variant"=w66) -> ("String Array"=w64:string[])  [unwired: 8 in]
      n16 = call-poly "Variant to Data.vi"("Variant"=w75) -> ("String"=w73:string)  [unwired: 8 in]
      n17 = call "Show Animated Busy Icon with Message.vi"("Already active? (F)"=w58, "Message"=w57, "Error In"=w62, "Target VI Refnum"=w59) -> ("Error Out"=w61:errorcluster)  [unwired: 7 in]
      n18 = case shown="\"Edit Palette List...\"" w73 {
        selector: w73 -> [_ w99 _]
        tunnel: w74 -> [_ _ _]
        tunnel: [w81 w86 w113] -> w72
        tunnel: [w80 w92 w111] -> w70
        tunnel: ["Palette List Edited" ("Append to Message") _ _] -> w67
        tunnel: w64 -> [w77 w90 _]
        tunnel: w63 -> [w76 w85 _]
        tunnel: w61 -> [_ _ w109]
        frame "Edit Palette List..." {
          n19 = call "Edit Image Palette List Dialog.vi"("Palette List (in)"=w77) -> ("Palette List (out)"=w84:string[])  [unwired: 10 in]
          n20 = call "Alligator Variables Storage.vi"("Get(F)/Set"=TRUE, "AlliGator Variable"=w76, "Data in"=w84) -> ("Error Out"=w82:errorcluster)  [unwired: 6 in, 2 out]
          n21 = call "AlliGator Check Selected Palette.vi"("Error In"=w82, "Image"=AlliGator_Image_Display_Type."Decay Fit Parameter Map") -> ("Error Out"=w81:errorcluster, "Image Display Palette Information"=w80:T13)  [unwired: 8 in]
        }
        frame Default {
          n22 = call "Get User Palette Choice.vi"("Palette"=w99) -> ("Error Out"=w95:errorcluster, "Palette Colors"=w97:u32[], "Palette Type"=w98:T14, "Palette Name (# Colors)"=w88:string, "Interpolate?"=w93:bool, "Built-in Palette?"=w89:bool)  [unwired: 3 in, 2 out]
          n23 = Bundle(cluster=T13 {"Palette Name [# Colors,int?,inv?]"="", "Palette Type"=0, "Palette Colors"=[], "Interpolate?"=FALSE} ("Image Display Palette Information"), "Palette Name [# Colors,int?,inv?]"=w88, "Palette Type"=w98, "Palette Colors"=w97, "Interpolate?"=w93) -> (w92:T13)
          n24 = call "Alligator Variables Storage.vi"("Get(F)/Set"=TRUE, "AlliGator Variable"=AlliGator_Variables_List."Decay Fit Parameter Map:Palette Information" ("Alligator Variable"), "Error In"=w95, "Data in"=w92) -> ("Error Out"=w87:errorcluster)  [unwired: 5 in, 2 out]
          n25 = case shown="False" w89 {
            tunnel: w87 -> [w107 w108]
            tunnel: [w106 w108] -> w86
            tunnel: w88 -> [w105 _]
            tunnel: w90 -> [w104 _]
            tunnel: w85 -> [w100 _]
            frame False {
              n26 = Build Array (concatenate)(w104, w105) -> (w103:string[])
              n27 = call-poly <userlib>:"Remove Duplicates from 1D Array__ogtk.vi"("Input Array"=w103) -> ("Output Array"=w102:string[])  [unwired: 1 out]
              n28 = call "Alligator Variables Storage.vi"("Get(F)/Set"=TRUE, "AlliGator Variable"=w100, "Error In"=w107, "Data in"=w102) -> ("Error Out"=w106:errorcluster)  [unwired: 5 in, 2 out]
            }
            frame True {
            }
          }
        }
        frame "Refresh Image" {
          n29 = call "Alligator Variables Storage.vi"("Get(F)/Set"=FALSE, "AlliGator Variable"=AlliGator_Variables_List."Decay Fit Parameter Map:Palette Information" ("Alligator Variable"), "Error In"=w109) -> ("Error Out"=w114:errorcluster, "Data out"=w115:variant)  [unwired: 6 in, 1 out]
          n30 = Variant To Data(error in=w114, type=T13 {"Palette Name [# Colors,int?,inv?]"="", "Palette Type"=0, "Palette Colors"=[], "Interpolate?"=FALSE} ("Image Display Palette Information"), Variant=w115) -> (data=w111:T13, error out=w113:errorcluster)
        }
      }
      n31 = call "AlliGator Update Decay Fit Parameter Map Palette.vi"("error in (no error)"=w72, "Decay Fit Parameter Map Display Palette Information"=w70, "Decay Fit Map Ctrl Refums"=w56) -> ("error out"=w68:errorcluster)  [unwired: 8 in]
      n32 = call "Hide Animated Busy Icon with Message.vi"("Already active? (F)"=w58, "Error In"=w68, "Target VI reference"=w59) -> ("Error Out"=w60:errorcluster)  [unwired: 8 in]
    }
    frame "Decay Fit Parameter Map:Change Map Resolution" {
      w125 = TRUE ("Get(F)/Set")
      w138 = TRUE  # Parameter changed
      w124 = AlliGator_Variables_List."Decay Fit Parameter Map:Y Resolution" ("Alligator Variable")
      w128 = AlliGator_Variables_List."Decay Fit Parameter Map:X Resolution" ("Alligator Variable")
      n33 = call "Alligator Variables Storage.vi"("AlliGator Variable"=w128, "Error In"=w143) -> ("Error Out"=w119:errorcluster, "Data out"=w147:variant)  [unwired: 7 in, 1 out]
      n34 = call-poly "Variant to Data.vi"("Variant"=w147) -> ("Value"=w146:i32)  [unwired: 8 in]
      n35 = call "Alligator Variables Storage.vi"("AlliGator Variable"=w124, "Error In"=w119) -> ("Error Out"=w144:errorcluster, "Data out"=w148:variant)  [unwired: 7 in, 1 out]
      n36 = call-poly "Variant to Data.vi"("Variant"=w148) -> ("Value"=w145:i32)  [unwired: 8 in]
      n37 = property class="Enum (strict)"(reference=w120, error in=w119) -> (error out=w117:errorcluster, "Value"=w134:T17)  [unwired: 1 out]
      n38 = call "AlliGator Decay Fit Parameter Map Size Dialog.vi"("error in (no error)"=w144, "Y Resolution"=w145, "X Resolution"=w146, "Message"="Enter the original dataset's X and Y resolution:") -> ("error out"=w129:errorcluster, "Y Resolution"=w122:i32, "X Resolution"=w127:i32)  [unwired: 4 in, 1 out]
      n39 = Bundle(cluster=T16 {"Parameter"=enum."Offset", "Parameter changed"=FALSE} ("output cluster"), "Parameter"=w134, "Parameter changed"=w138) -> (w136:T16)
      n40 = call "Alligator Variables Storage.vi"("Get(F)/Set"=w125, "AlliGator Variable"=w128, "Error In"=w129, "Data in"=w127) -> ("Error Out"=w126:errorcluster)  [unwired: 5 in, 2 out]
      n41 = Bundle By Name(cluster=T6 {"AlliGator Q Event"=enum."Decay Fit Parameter Map:Build Decay Fit Parameter Map", "Data"=variant} ("Alligator Atomic Action"), "Data"=w136) -> (w137:T6)
      n42 = call "Alligator Variables Storage.vi"("Get(F)/Set"=w125, "AlliGator Variable"=w124, "Error In"=w126, "Data in"=w122) -> ("Error Out"=w123:errorcluster)  [unwired: 5 in, 2 out]
      n43 = Merge Errors(w117, w123) -> (w118:errorcluster)
      n44 = call-poly "AlliGator Add Action(s) to Stack.vi"("Elements Order in Action Stack (Default: 2 BEFORE 1)"=Alligator_Elements_Order_in_Action_Stack."Enqueue 2 BEFORE 1", "Error In"=w118, "Alligator Atomic Action"=w137, "Alligator Queue Element 1"=w142) -> ("Error Out"=w133:errorcluster, "Alligator Queue Element 1 (+ 2)"=w141:T6[])  [unwired: 6 in]
      n45 = Format Into String(format string="New Decay Fit Parameter Map Resolution:\nX Resolution: %d\nY Resolution: %d", error in=w133, w127, w122) -> (resulting string=w130:string, error out=w132:errorcluster)  [unwired: 1 in]
    }
    frame "Decay Fit Parameter Map:Display Range Mouse Move" {
      # "\"Decay Fit Parameter Map:Display Range Mouse Move\""
      n46 = call "Extend Display Range to Match Slider(s).vi"("error in (no error)"=w154, "Display Range"=w152) -> ("error out"=w153:errorcluster)  [unwired: 7 in, 2 out]
      n47 = Variant To Data(error in=w153, Variant=w157) -> (data=w155:T17, error out=w156:errorcluster)  [unwired: 1 in]
      n48 = call "AlliGator Decay Fit Parameter Map Range Mouse Move Event.vi"("Error In"=w156, "Decay Fit Parameter"=w155, "AlliGator Actions in"=w160) -> ("Error Out"=w158:errorcluster, "AlliGator Actions out"=w159:T6[])  [unwired: 7 in]
    }
    frame "Decay Fit Parameter Map:Export All Decay Fit Parameter Maps Data as ASCII" {
      # "\"Export All Decay Fit Parameter Maps Data as ASCII\""
      n49 = call "Show Animated Busy Icon with Message.vi"("Already active? (F)"=w165, "Message"=w171, "Error In"=w163, "Target VI Refnum"=w170) -> ("Error Out"=w166:errorcluster)  [unwired: 7 in]
      n50 = call "AlliGator Save All Decay Fit Parameter Maps to ASCII.vi"("error in (no error)"=w166, "Data Value Reference in"=w168) -> ("error out"=w167:errorcluster, "Data Value Reference out"=w169:refnum<data-value>, "Message"=w164:string)  [unwired: 7 in]
      n51 = call "Hide Animated Busy Icon with Message.vi"("Already active? (F)"=w165, "Error In"=w167, "Target VI reference"=w170) -> ("Error Out"=w172:errorcluster)  [unwired: 8 in]
    }
    frame "Decay Fit Parameter Map:Export Decay Fit Parameter Map Data as ASCII" {
      # "\"Export Decay Fit Parameter Map Data as ASCII\""
      n52 = call-poly "Variant to Data.vi"("Variant"=w188) -> ("Value"=w187:bool)  [unwired: 8 in]
      n53 = property class="Enum (strict)"(reference=w175, error in=w174) -> (error out=w176:errorcluster, "Value"=w184:T29)  [unwired: 1 out]
      n54 = call "Show Animated Busy Icon with Message.vi"("Already active? (F)"=w178, "Message"=w185, "Error In"=w176, "Target VI Refnum"=w183) -> ("Error Out"=w180:errorcluster)  [unwired: 7 in]
      n55 = call "AlliGator Save Decay Fit Parameter Map to ASCII.vi"("Fit Parameter"=w184, "error in (no error)"=w180, "Dialog?"=w187, "Data Value Reference in"=w181) -> ("error out"=w179:errorcluster, "Data Value Reference out"=w182:refnum<data-value>, "Message"=w177:string)  [unwired: 5 in]
      n56 = call "Hide Animated Busy Icon with Message.vi"("Already active? (F)"=w178, "Error In"=w179, "Target VI reference"=w183) -> ("Error Out"=w186:errorcluster)  [unwired: 8 in]
    }
    frame "Decay Fit Parameter Map:Export ROI NLSF Data as ASCII" {
      n57 = call-poly "Variant to Data.vi"("Variant"=w201) -> ("Value"=w198:bool)  [unwired: 8 in]
      n58 = call "Show Animated Busy Icon with Message.vi"("Already active? (F)"=w191, "Message"=w194, "Error In"=w190, "Target VI Refnum"=w192) -> ("Error Out"=w195:errorcluster)  [unwired: 7 in]
      n59 = call "AlliGator Export ROI(s) NLSF Parameters as ASCII File.vi"("error in (no error)"=w195, "All ROIs"=w198, "AlliGator IV DVR in"=w200) -> ("error out"=w197:errorcluster, "Message"=w196:string, "AlliGator IV DVR out"=w199:refnum<data-value>)  [unwired: 6 in]
      n60 = call "Hide Animated Busy Icon with Message.vi"("Already active? (F)"=w191, "Error In"=w197, "Target VI reference"=w192) -> ("Error Out"=w193:errorcluster)  [unwired: 8 in]
    }
    frame "Decay Fit Parameter Map:Fit Result Constraints Window" {
      n61 = call "AlliGator Get Ancillary Window Path.vi"("Error In"=w204, "AlliGator Window"=AlliGator_Windows_List."Fit Result Constraints Window" ("AlliGator Windows")) -> ("Error Out"=w207:errorcluster, "VI Path"=w208:path)  [unwired: 8 in]
      n62 = call "Run Vi.vi"("VI Path"=w208, "error in (no error)"=w207, "Start Hidden? (F)"=TRUE) -> ("error out"=w203:errorcluster)  [unwired: 5 in, 1 out]
    }
    frame "Decay Fit Parameter Map:Mouse Move" {
      # "\"Decay Fit Parameter Map:Mouse Move\""
      n63 = call "AlliGator Display Current Decay Fit Parameter Map (X,Y, I).vi"("error in (no error)"=w217, "AlliGator Internal Variables DVR"=w216) -> ("error out"=w213:errorcluster, "AlliGator Internal Variables DVR"=w215:refnum<data-value>)  [unwired: 8 in]
      n64 = flat-sequence {
        tunnel: w214 -> [w222]
        tunnel: w213 -> [w221]
        tunnel: [w221] -> w212
        frame #0 {
          n65 = call "AlliGator Generic Image Display Mouse Move Flag.vi"("Image Control Refnum"=w222, "Flag (in)"=FALSE, "Read/Write"=Read-Write."Write") -> ()  [unwired: 6 in, 1 out]
        }
      }
    }
    frame "Decay Fit Parameter Map:Mouse Up" {
      # "\"Decay Fit Parameter Map:Mouse Up\""
      n66 = Variant To Data(error in=w224, type=T20 {"Current ROI Tool"=8, "ROI Descriptor"={"Global Rectangle"=[], "Contours"=[]}, "Shift"=FALSE, "Alt"=FALSE, "Image Display Refnum"=refnum} ("Phasor Plot Mouse Up Event Data"), Variant=w228) -> (data=w227:T20, error out=w226:errorcluster)
      n67 = call "AlliGator Decay Fit Parameter Map Mouse Up Event.vi"("error in (no error)"=w226, "Image Mouse Up Event Data"=w227, "AlliGator Actions in"=w231) -> ("error out"=w229:errorcluster, "AlliGator Actions out"=w230:T6[])  [unwired: 7 in]
    }
    frame "Decay Fit Parameter Map:Overlay Decay Fit Parameter Map in Source Image" {
      # "\"Overlay Decay Fit Parameter Map in Source Image\""
      n68 = property class="Bool (strict)"(reference=w237, error in=w236) -> (error out=w241:errorcluster, "Value"=w251:bool)  [unwired: 1 out]
      n69 = call "Show Animated Busy Icon with Message.vi"("Already active? (F)"=w243, "Message"=w242, "Error In"=w241, "Target VI Refnum"=w244) -> ("Error Out"=w250:errorcluster)  [unwired: 7 in]
      n70 = call "AlliGator Overlay Decay Fit Parameter Map in Original Image.vi"("Decay Fit Parameter Map Color Scale Refnum"=w238, "Image Color Scale Refnum"=w235, "Error In"=w250, "Destination Image Control Refnum"=w234, "AlliGator IV DVR in"=w248) -> ("Error Out"=w249:errorcluster, "AlliGator IV DVR out"=w247:refnum<data-value>)  [unwired: 4 in, 1 out]
      n71 = call "Hide Animated Busy Icon with Message.vi"("Already active? (F)"=w243, "Error In"=w249, "Target VI reference"=w244) -> ("Error Out"=w240:errorcluster)  [unwired: 8 in]
      n72 = case shown="True" w251 {
        tunnel: w246 -> [w253 w259]
        tunnel: [w253 w256] -> w245
        tunnel: w240 -> [w252 w255]
        tunnel: [w252 w254] -> w239
        frame False {
        }
        frame True {
          n73 = call-poly "AlliGator Add Action(s) to Stack.vi"("Elements Order in Action Stack (Default: 2 BEFORE 1)"=Alligator_Elements_Order_in_Action_Stack."Enqueue 2 BEFORE 1", "Error In"=w255, "Alligator Atomic Action"=T6 {"AlliGator Q Event"=enum."Image:Save Displayed Image with Overlay", "Data"=variant}, "Alligator Queue Element 1"=w259) -> ("Error Out"=w254:errorcluster, "Alligator Queue Element 1 (+ 2)"=w256:T6[])  [unwired: 6 in]
        }
      }
    }
    frame "Decay Fit Parameter Map:Parameter 2 vs Parameter 1 Scatterplot" {
      # "Parameter 2 vs Parameter 1 Scatterplot"
      n74 = call "Show Animated Busy Icon with Message.vi"("Already active? (F)"=w276, "Message"=w280, "Error In"=w260, "Target VI Refnum"=w279) -> ("Error Out"=w274:errorcluster)  [unwired: 7 in]
      n75 = Variant To Data(error in=w274, type=T26 {"Fit Parameter 1"=enum."Offset", "Fit Parameter 2"=enum."Offset"}, Variant=w275) -> (data=w272:T26, error out=w268:errorcluster)
      n76 = Unbundle By Name(w272) -> ("Fit Parameter 1"=w271:T17, "Fit Parameter 2"=w270:T17)
      n77 = call "AlliGator Apply Fit Result Constraints.vi"("error in (no error)"=w268, "AlliGator IV DVR in"=w266) -> ("error out"=w267:errorcluster, "Message"=w263:string, "AlliGator IV DVR out"=w265:refnum<data-value>)  [unwired: 7 in]
      n78 = call "AlliGator Plot Fit Parameter 2 vs Parameter 1.vi"("error in (no error)"=w267, "Fit Parameter 2"=w270, "Fit Parameter 1"=w271, "Data Value Reference in"=w265) -> ("error out"=w277:errorcluster, "Data Value Reference out"=w278:refnum<data-value>, "Message"=w269:string)  [unwired: 5 in]
      n79 = Concatenate Strings(w263, "\r\n", w269) -> (w264:string)
      n80 = call "Hide Animated Busy Icon with Message.vi"("Already active? (F)"=w276, "Error In"=w277, "Target VI reference"=w279) -> ("Error Out"=w281:errorcluster)  [unwired: 8 in]
    }
    frame "Decay Fit Parameter Map:Python Function Decay Fit Parameters Map Event" {
      # "\"Decay Fit Parameters:Python Function Decay Fit Parameters Map Event\""
      n81 = One Button Dialog(message="Not yet supported....") -> ()  [unwired: 1 in, 1 out]
      n82 = call "Play Error Sound.vi"() -> ()  [unwired: 27 in, 1 out]
    }
    frame "Decay Fit Parameter Map:Save Decay Fit Parameter Map Image" {
      # "\"Save Decay Fit Parameter Map Image\""
      n83 = call-poly "Variant to Data.vi"("Variant"=w303) -> ("Value"=w297:bool)  [unwired: 8 in]
      n84 = property class="Enum (strict)"(reference=w289, error in=w288) -> (error out=w296:errorcluster, "Value"=w298:T29)  [unwired: 1 out]
      n85 = call "Show Animated Busy Icon with Message.vi"("Already active? (F)"=w291, "Message"=w294, "Error In"=w296, "Target VI Refnum"=w292) -> ("Error Out"=w295:errorcluster)  [unwired: 7 in]
      n86 = call "AlliGator Save Decay Fit Parameter Map Image.vi"("Dialog?"=w297, "error in (no error)"=w295, "Fit Parameter"=w298, "Image Control Refnum"=w290, "IV DVR"=w302) -> ("error out"=w299:errorcluster, "Message"=w300:string, "IV DVR"=w301:refnum<data-value>)  [unwired: 4 in]
      n87 = call "Hide Animated Busy Icon with Message.vi"("Already active? (F)"=w291, "Error In"=w299, "Target VI reference"=w292) -> ("Error Out"=w293:errorcluster)  [unwired: 8 in]
    }
    frame "Decay Fit Parameter Map:Save-Load IRFs & Fit Data" {
      # "\"Save-Load IRFs & Fit Data\""
      n88 = Variant To Data(error in=w305, type=T27 {"Load/Save"=FALSE, "File Path"=path ""} ("Calibration File Information"), Variant=w318) -> (data=w316:T27, error out=w306:errorcluster)
      n89 = Unbundle By Name(w316) -> ("File Path"=w315:path, "Load/Save"=w314:bool)
      n90 = call "Show Animated Busy Icon with Message.vi"("Already active? (F)"=w308, "Message"=w319, "Error In"=w306, "Target VI Refnum"=w313) -> ("Error Out"=w310:errorcluster)  [unwired: 7 in]
      n91 = call "AlliGator Save-Load IRFs & Fit Data (Map).vi"("error in (no error)"=w310, "Write(T)/Load (F)"=w314, "File Path"=w315, "Data Value Reference in"=w311) -> ("error out"=w309:errorcluster, "Data Value Reference out"=w312:refnum<data-value>, "Message"=w307:string)  [unwired: 5 in]
      n92 = call "Hide Animated Busy Icon with Message.vi"("Already active? (F)"=w308, "Error In"=w309, "Target VI reference"=w313) -> ("Error Out"=w320:errorcluster)  [unwired: 8 in]
    }
    frame "Decay Fit Parameter Map:Selected Parameter Scatterplot" {
      # "Selected Parameter Scatterplot"
      n93 = call-poly "Variant to Data.vi"("Variant"=w339) -> ("Value"=w338:i32)  [unwired: 8 in]
      n94 = property class="Enum (strict)"(reference=w322) -> (error out=w331:errorcluster, "Value"=w336:T29)  [unwired: 1 in, 1 out]
      n95 = call "Show Animated Busy Icon with Message.vi"("Already active? (F)"=w333, "Message"=w340, "Error In"=w331, "Target VI Refnum"=w337) -> ("Error Out"=w330:errorcluster)  [unwired: 7 in]
      n96 = call "AlliGator Apply Fit Result Constraints.vi"("error in (no error)"=w330, "AlliGator IV DVR in"=w329) -> ("error out"=w328:errorcluster, "Message"=w325:string, "AlliGator IV DVR out"=w327:refnum<data-value>)  [unwired: 7 in]
      n97 = call "AlliGator Plot Fit Parameter Scatterplot.vi"("Fit Parameter"=w336, "error in (no error)"=w328, "ROI idx (2147483647: all ROIs)"=w338, "Data Value Reference in"=w327) -> ("error out"=w334:errorcluster, "Data Value Reference out"=w335:refnum<data-value>, "Message"=w332:string)  [unwired: 5 in]
      n98 = Concatenate Strings(w325, "\r\n", w332) -> (w326:string)
      n99 = call "Hide Animated Busy Icon with Message.vi"("Already active? (F)"=w333, "Error In"=w334, "Target VI reference"=w337) -> ("Error Out"=w341:errorcluster)  [unwired: 8 in]
    }
    frame "Decay Fit Parameter Map:Selected Parameter vs Intensity Scatterplot" {
      # "Selected Parameter vs Intensity"
      n100 = call-poly "Variant to Data.vi"("Variant"=w361) -> ("Value"=w360:i32)  [unwired: 8 in]
      n101 = property class="Enum (strict)"(reference=w344, error in=w343) -> (error out=w353:errorcluster, "Value"=w358:T29)  [unwired: 1 out]
      n102 = call "Show Animated Busy Icon with Message.vi"("Already active? (F)"=w355, "Message"=w362, "Error In"=w353, "Target VI Refnum"=w359) -> ("Error Out"=w350:errorcluster)  [unwired: 7 in]
      n103 = call "AlliGator Apply Fit Result Constraints.vi"("error in (no error)"=w350, "AlliGator IV DVR in"=w352) -> ("error out"=w349:errorcluster, "Message"=w347:string, "AlliGator IV DVR out"=w351:refnum<data-value>)  [unwired: 7 in]
      n104 = call "AlliGator Plot Decay Fit Parameter vs Intensity Scatterplot v2.vi"("Fit Parameter"=w358, "error in (no error)"=w349, "ROI idx (2147483647: all ROIs)"=w360, "Data Value Reference in"=w351) -> ("error out"=w356:errorcluster, "Data Value Reference out"=w357:refnum<data-value>, "Message"=w354:string)  [unwired: 5 in]
      n105 = call "Hide Animated Busy Icon with Message.vi"("Already active? (F)"=w355, "Error In"=w356, "Target VI reference"=w359) -> ("Error Out"=w363:errorcluster)  [unwired: 8 in]
      n106 = Concatenate Strings(w347, "\r\n", w354) -> (w348:string)
    }
    frame "Decay Fit Parameter Map:Set Decay Fit Parameter Map Selection" {
      # "used in script"
      # "\"Decay Fit  Parameter Map:Set Decay Fit  Parameter Map Selection\""
      n107 = Variant To Data(error in=w365, type=Decay_Fit_Parameters_&_Derived_Quantities_List_v2."Offset" ("Fit Parameter"), Variant=w376) -> (data=w373:T17, error out=w372:errorcluster)
      n108 = property class="Enum (strict)"(reference=w366, error in=w372, "Value"=w373) -> (error out=w371:errorcluster)  [unwired: 1 out]
      n109 = Format Into String(format string="Decay Fit Parameter Map Selection set to %s", error in=w371, w373) -> (resulting string=w369:string, error out=w368:errorcluster)  [unwired: 1 in]
    }
    frame "Decay Fit Parameter Map:Update Local Decay Plots" {
      # "\"Update Local Decay Plots\""
      n110 = Variant To Data(error in=w378, Variant=w389) -> (data=w388:T30, error out=w385:errorcluster)  [unwired: 1 in]
      n111 = call "Show Animated Busy Icon with Message.vi"("Already active? (F)"=w380, "Message"=w379, "Error In"=w385, "Target VI Refnum"=w381) -> ("Error Out"=w383:errorcluster)  [unwired: 7 in]
      n112 = call "AlliGator Send Local Decay Plots.vi"("error in (no error)"=w383, "ROI Descriptor"=w388, "AlliGator IV DVR in"=w387) -> ("error out"=w384:errorcluster, "AlliGator IV DVR out"=w386:refnum<data-value>)  [unwired: 7 in]
      n113 = call "Hide Animated Busy Icon with Message.vi"("Already active? (F)"=w380, "Error In"=w384, "Target VI reference"=w381) -> ("Error Out"=w382:errorcluster)  [unwired: 8 in]
    }
    frame "Decay Fit Parameter Map:Variance Significance Maps" {
      n114 = call "AlliGator Enter CV Analysis Parameters Dialog.vi"("Error In"=w396) -> ("Error Out"=w399:errorcluster, "Cancelled?"=w397:bool, "Function Parameters out"=w400:T31)  [unwired: 8 in]
      n115 = case shown="False" w397 {
        tunnel: w405 -> [w426 w428]
        tunnel: w404 -> [w425 w429]
        tunnel: [w424 w429] -> w403
        tunnel: [w422 _] -> w402
        tunnel: [w421 w428] -> w401
        tunnel: w400 -> [w420 _]
        tunnel: w399 -> [w412 w427]
        tunnel: [w413 w427] -> w395
        tunnel: w394 -> [w409 _]
        tunnel: w393 -> [w408 _]
        tunnel: w392 -> [w407 _]
        tunnel: w391 -> [w406 _]
        frame False {
          n116 = call "Show Animated Busy Icon with Message.vi"("Already active? (F)"=w408, "Message"=w407, "Error In"=w412, "Target VI Refnum"=w409) -> ("Error Out"=w411:errorcluster)  [unwired: 7 in]
          n117 = call "AlliGator Lifetime Variance Maps Calculation.vi"("error in (no error)"=w411, "Function Parameters"=w420, "Decay Fit Parameter"=w406, "AlliGator IV DVR in"=w426) -> ("error out"=w410:errorcluster, "Parameter Map Names"=w416:string[], "New Parameter Set Name"=w417:string, "AlliGator IV DVR out"=w421:refnum<data-value>, "Message"=w422:string)  [unwired: 3 in]
          n118 = Bundle By Name(cluster=T28 {"New Parameter Set Name"="", "Parameter Map Names"=[]} ("output cluster"), "New Parameter Set Name"=w417, "Parameter Map Names"=w416) -> (w415:T28)
          n119 = Bundle By Name(cluster=T6 {"AlliGator Q Event"=enum."Parameter Map:Add Parameter Map Set", "Data"=variant} ("Alligator Atomic Action"), "Data"=w415) -> (w418:T6)
          n120 = call "Hide Animated Busy Icon with Message.vi"("Already active? (F)"=w408, "Error In"=w410, "Target VI reference"=w409) -> ()  [unwired: 8 in, 1 out]
          n121 = call-poly "AlliGator Add Action(s) to Stack.vi"("Elements Order in Action Stack (Default: 2 BEFORE 1)"=Alligator_Elements_Order_in_Action_Stack."Enqueue 2 BEFORE 1", "Error In"=w410, "Alligator Atomic Action"=w418, "Alligator Queue Element 1"=w425) -> ("Error Out"=w413:errorcluster, "Alligator Queue Element 1 (+ 2)"=w424:T6[])  [unwired: 6 in]
        }
        frame True {
        }
      }
    }
    frame "Decay Fit Parameter Map:Use ROI" {
      # "Decay Fit Parameter Map:Use ROI"
      n122 = Variant To Data(error in=w433, type=T21 {"Global Rectangle"=[], "Contours"=[]} ("ROI Descriptor"), Variant=w434) -> (data=w431:T21, error out=w436:errorcluster)
      n123 = property class="ImageControl"(reference=w430, error in=w436, "ROI"=w431) -> (error out=w432:errorcluster)  [unwired: 1 out]
    }
  }
  "Data Value Reference out" <- w29
  "error out" <- w14
  "AlliGator Q Elements out" <- w24
  "Script out" <- w21
  n124 = call "Get Current Message Text Format.vi"("Text Format"=w16) -> ("Error Out"=w15:errorcluster, "Message Formatting"=w18:T2)  [unwired: 8 in]
  n125 = call "AlliGator Package Notebook Messages.vi"("Error In"=w15, "Message Formatting"=w18, "Message"=w19, "AlliGator Q Event in"="AlliGator Q Event in") -> ("[Notebook Message]"=→"[Notebook Message]":T1[])  [unwired: 6 in, 1 out]
